vi "ConvertTextBasedCodeToLabVIEW.vi"() -> ()   [LabVIEW 2020]
uses:
  String/GDSString_ClassDescriptionType.ctl
  String/GDSString_AccessScopeModifierType.ctl
  String/GDSString_ModifierType.ctl
  String/GDSString_MethodDescriptionType.ctl
  CommonVIs/CommonVIs_AttributeType.ctl
  CommonVIs/CommonVIs_AttributeDataType.ctl
  CommonVIs/CommonVIs_PropertyType.ctl
  String/GDSString_ClassParentType.ctl
  String/GDSString_ClassType.ctl
  String/GDSString_ClassOwnerType.ctl
  CommonVIs/CommonVIs_EnumType.ctl
  CommonVIs/CommonVIs_StructType.ctl
  API/GDSAPI_SubVIs/GDSAPI_PropertyMethodType.ctl
  ScriptingFunctions/Scripting_ConnectorPanePatternType.ctl
  ConvertTextToLv_SubVIs/ConvertTextBasedCodeToLabVIEW_MissingType.ctl
  ConvertTextToLv_SubVIs/ConvertTextBasedCodeToLabVIEW_MissingTypeIconType.ctl
  <vilib>/picture/picture.llb/imagedata.ctl
  <vilib>/Utility/miscctls.llb/LVFontTypeDef.ctl
  <vilib>/Utility/miscctls.llb/LVBoundsTypeDef.ctl
  ConvertTextToLv_SubVIs/ConvertTextBasedCodeToLabVIEW_CreateClassesOption.ctl
  API/GDSAPI_SubVIs/GDSAPI_ClassProviderType.ctl
  <vilib>/Utility/miscctls.llb/LVPositionTypeDef.ctl
  <vilib>/Platform/browser.llb/Open URL in Default Browser (path).vi
  <vilib>/Utility/miscctls.llb/LVPointTypeDef.ctl
panel:
  out "Classes":T1[](array[typedef])
  out "Tab":T13(tab)
  in  "RemoveSelectedFiles":bool
  in  "ClearList":bool
  in  "FileList":i32[](listbox) caption="File List"
  in  "CopyfromClipboard":bool
  in  "Code":string caption="Java or C# Code"
  in  "Path":path caption="Java or C# File or top level folder"
  out "FileListText":bool
  in  "Ring":u16(ring)=2 items=["Select action to handle missing type", "Create stub code as class", "Create stub code as interface", "Remove dependency to this type"]
  out "Picture":picture caption="Missing Classes and types"
  in  "ExistingClasses":path
  out "MissingText1":string
  out "MissingText2":string
  in  "BetterNames":bool
  in  "ViewClassOverView":bool
  in  "ClassType":T14(ring) caption="Class Type"
  in  "Top Folder for all classes":path caption="Folder will be created"
  in  "PropertyMethodType":T15 caption="Property Method Type"
  in  "VI/Method Pattern type":T16 items=["4x4x4", "5x6x5", "6x8x6"]
  out "ProgressText":string
  in  "Previous":bool
  in  "Cancel":bool
  in  "Next":bool
  out "error IO":errorcluster
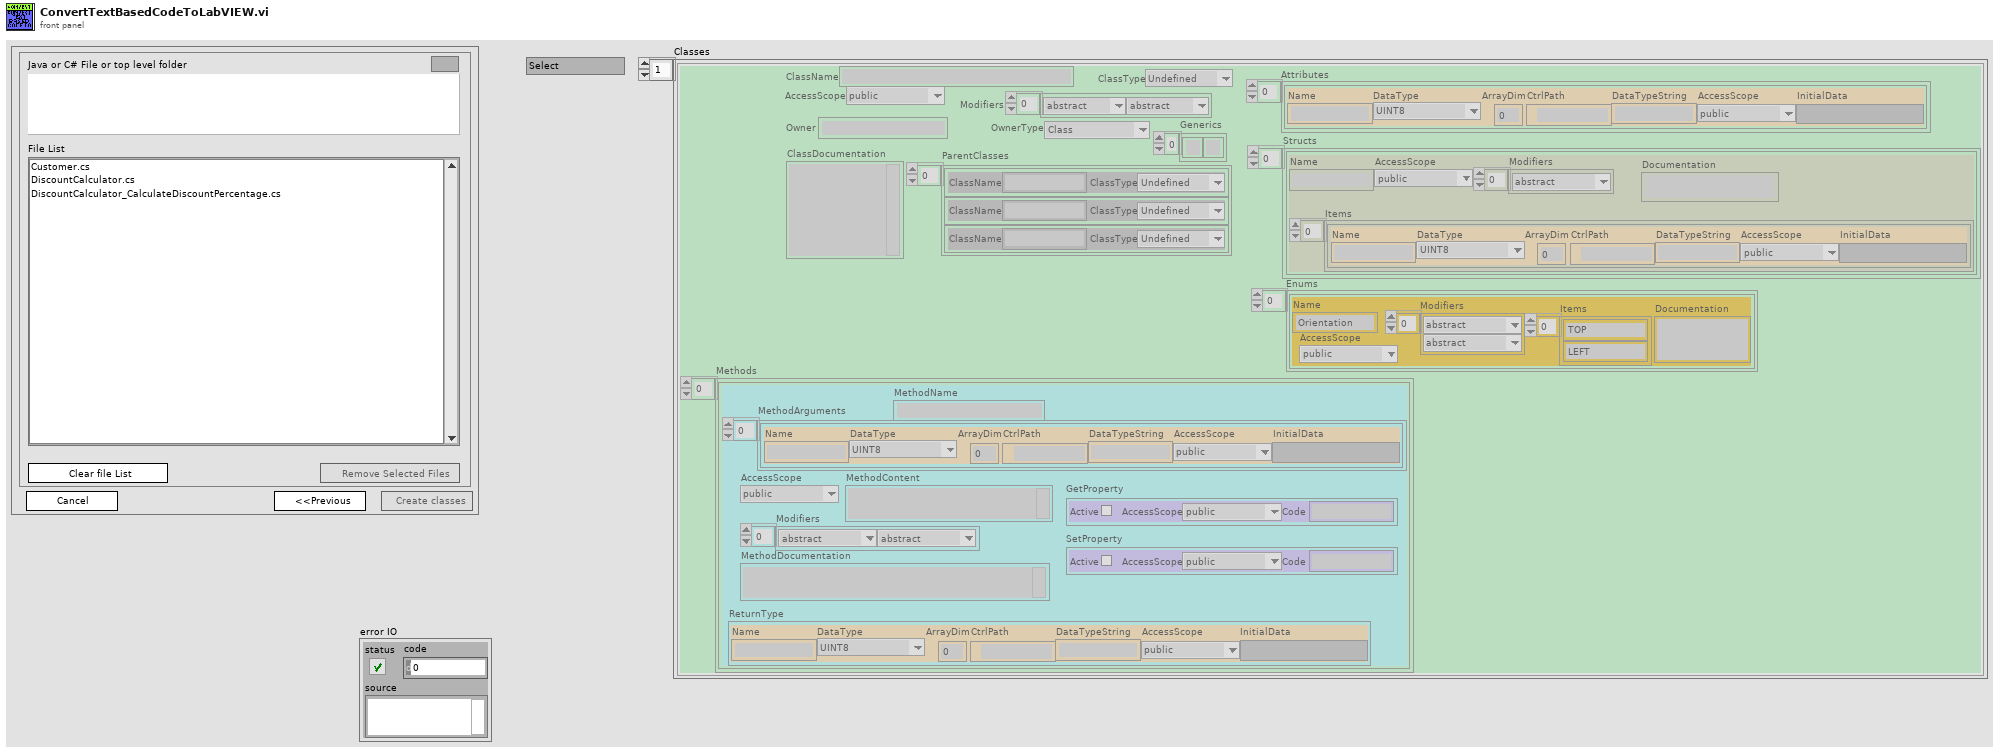
[diagram p1: front panel]
types:
  T1 = typedef "GDSString_ClassDescriptionType.ctl" = cluster{"ClassName":string, "AccessScope":T2, "Modifiers":T3[], "ClassDocumentation":string, "Methods":T4[], "ParentClasses":T8[], "ClassType":T9, "Owner":string, "OwnerType":T10, "Generics":string[], "Attributes":T5[], "Enums":T11[], "Structs":T12[]}
  T2 = typedef "GDSString_AccessScopeModifierType.ctl" = enum16{"public", "private", "protected", "internal"}
  T3 = typedef "GDSString_ModifierType.ctl" = enum16{"abstract", "static", "final", "synchronized", "strictfp", "async", "const", "event", "extern", "new", "native ", "override", "partial", "readonly", "sealed", "unsafe", "virtual", "volatile"}
  T4 = typedef "GDSString_MethodDescriptionType.ctl" = cluster{"ReturnType":T5, "MethodName":string, "AccessScope":T2, "Modifiers":T3[], "MethodDocumentation":string, "MethodContent":string, "MethodArguments":T5[], "GetProperty":T7, "SetProperty":T7}
  T5 = typedef "CommonVIs_AttributeType.ctl" = cluster{"Name":string, "DataType":T6, "ArrayDim":i32, "CtrlPath":path, "DataTypeString":string, "AccessScope":T2, "InitialData":variant}
  T6 = typedef "CommonVIs_AttributeDataType.ctl" = enum16{"UINT8", "INT8", "UINT16", "INT16", "UINT32", "INT32", "UINT64", "INT64", "SGL", "DBL", "EXT", "CSG", "CDB", "CXT", "TimeStamp", "STRING", "PATH", "BOOL", "ENUM", "RefNum", "VIRefNum", "LabVIEW Class", "Cluster", "Variant", "TypeDef", "Waveform", "LabVIEW Object", "Other", "void", "Set", "Map"}
  T7 = typedef "CommonVIs_PropertyType.ctl" = cluster{"Active":bool, "AccessScope":T2, "Code":string}
  T8 = typedef "GDSString_ClassParentType.ctl" = cluster{"ClassName":string, "ClassType":T9}
  T9 = typedef "GDSString_ClassType.ctl" = enum16{"Undefined", "Class", "Interface"}
  T10 = typedef "GDSString_ClassOwnerType.ctl" = enum16{"NoOwner", "Class", "Package/NameSpace"}
  T11 = typedef "CommonVIs_EnumType.ctl" = cluster{"Name":string, "AccessScope":T2, "Modifiers":T3[], "Items":string[], "Documentation":string}
  T12 = typedef "CommonVIs_StructType.ctl" = cluster{"Name":string, "AccessScope":T2, "Modifiers":T3[], "Items":T5[], "Documentation":string}
  T13 = enum32{"Select", "Analysing", "Missing", "Overview", "Working"}
  T14 = enum16{"Native By Value LabVIEW Classes", "Reference Object DVR (GOOP4)", "Reference Object  (GOOP3)"}
  T15 = typedef "GDSAPI_PropertyMethodType.ctl" = enum16{"PropertyMethod", "PropertyNode"}
  T16 = typedef "Scripting_ConnectorPanePatternType.ctl" = u16
  T17 = typedef "imagedata.ctl" = cluster{"image type":i32, "image depth":i32, "image":u8[], "mask":u8[], "colors":u32[], "Rectangle":cluster{"left":i16, "top":i16, "right":i16, "bottom":i16}}
  T18 = typedef "ConvertTextBasedCodeToLabVIEW_MissingType.ctl" = cluster{"Item":string, "Options":string[], "Icons":T19[], "Index":i32}
  T19 = typedef "ConvertTextBasedCodeToLabVIEW_MissingTypeIconType.ctl" = enum16{"?", "Add", "Delete", "Implement", "Inherit"}
  T20 = cluster{"Counter":i32, "Text":string, "Cancelled":bool, "Files":path[], "Classes":T1[], "MissingTypes":cluster{"ShowRing":bool, "Rectangle":cluster{"left":i16, "top":i16, "right":i16, "bottom":i16}, "IndexOffset":i32, "Row":i32, "Y-Distance":i32, "Selected":i32[], "Font":enum16{"User-specified Font", "Application Font", "System Font", "Dialog Font"}, "UserFont":cluster{"Font Name:":string, "Size":i16, "Strikeout?":bool, "Italic?":bool, "Underline?":bool, "Outline?":bool, "Shadow?":bool, "Bold?":bool}, "VerGap":i32, "HorGap":i32, "XStart2":i32, "XStart1":i32, "Rectangles":cluster{"left":i16, "top":i16, "right":i16, "bottom":i16}[], "VerticalRows":i32, "YStart":i32}, "MissingItems":T18[], "ExistingClassesFolders":path[], "StructsOusideClass":T12[], "EnumsOusideClass":T11[], "InterfaceItems":T18[], "Interface":bool, "MissingTypeSelected":i32[], "InterfaceSelected":i32[]}
  T21 = typedef "LVPointTypeDef.ctl" = cluster{"Horizontal":i16, "Vertical":i16}
  T22 = enum8{"Enabled", "Disabled", "Disabled and Grayed Out"}
  T23 = enum32{"Select", "Analysing", "Missing", "Overview"}
  T24 = typedef "LVFontTypeDef.ctl" = cluster{"Font Name":string, "Size":u16, "Bold":bool, "Italic":bool, "Underline":bool, "Strikeout":bool, "Color":u32}
  T25 = cluster{"left":i16, "top":i16, "right":i16, "bottom":i16}
  T26 = typedef "LVBoundsTypeDef.ctl" = cluster{"Width":u32, "Height":u32}
  T27 = typedef "ConvertTextBasedCodeToLabVIEW_CreateClassesOption.ctl" = cluster{"ClassProvider":T28, "PropertyMethodType":T15, "Pattern type":T16}
  T28 = typedef "GDSAPI_ClassProviderType.ctl" = enum16{"LabVIEW Native(By value)", "GOOP-3(By reference)", "GOOP-4(By reference)"}
  T29 = typedef "LVMouseTypeDef.ctl" = cluster{"Mouse Position":cluster{"X":i32, "Y":i32}, "Mouse Modifiers":cluster{"Button Down":bool, "Shift Mod":bool, "Menu Mod":bool, "Option Mod":bool}}
  T30 = cluster{"left":i16, "top":i16, "right":i16, "bottom":i16}[]
  T31 = cluster{"Font Name:":string, "Size":i16, "Strikeout?":bool, "Italic?":bool, "Underline?":bool, "Outline?":bool, "Shadow?":bool, "Bold?":bool}
  T32 = enum16{"User-specified Font", "Application Font", "System Font", "Dialog Font"}
  T33 = typedef "LVRectTypeDef.ctl" = cluster{"Left":i16, "Top":i16, "Right":i16, "Bottom":i16}
  T34 = typedef "LVPositionTypeDef.ctl" = cluster{"Left":i32, "Top":i32}
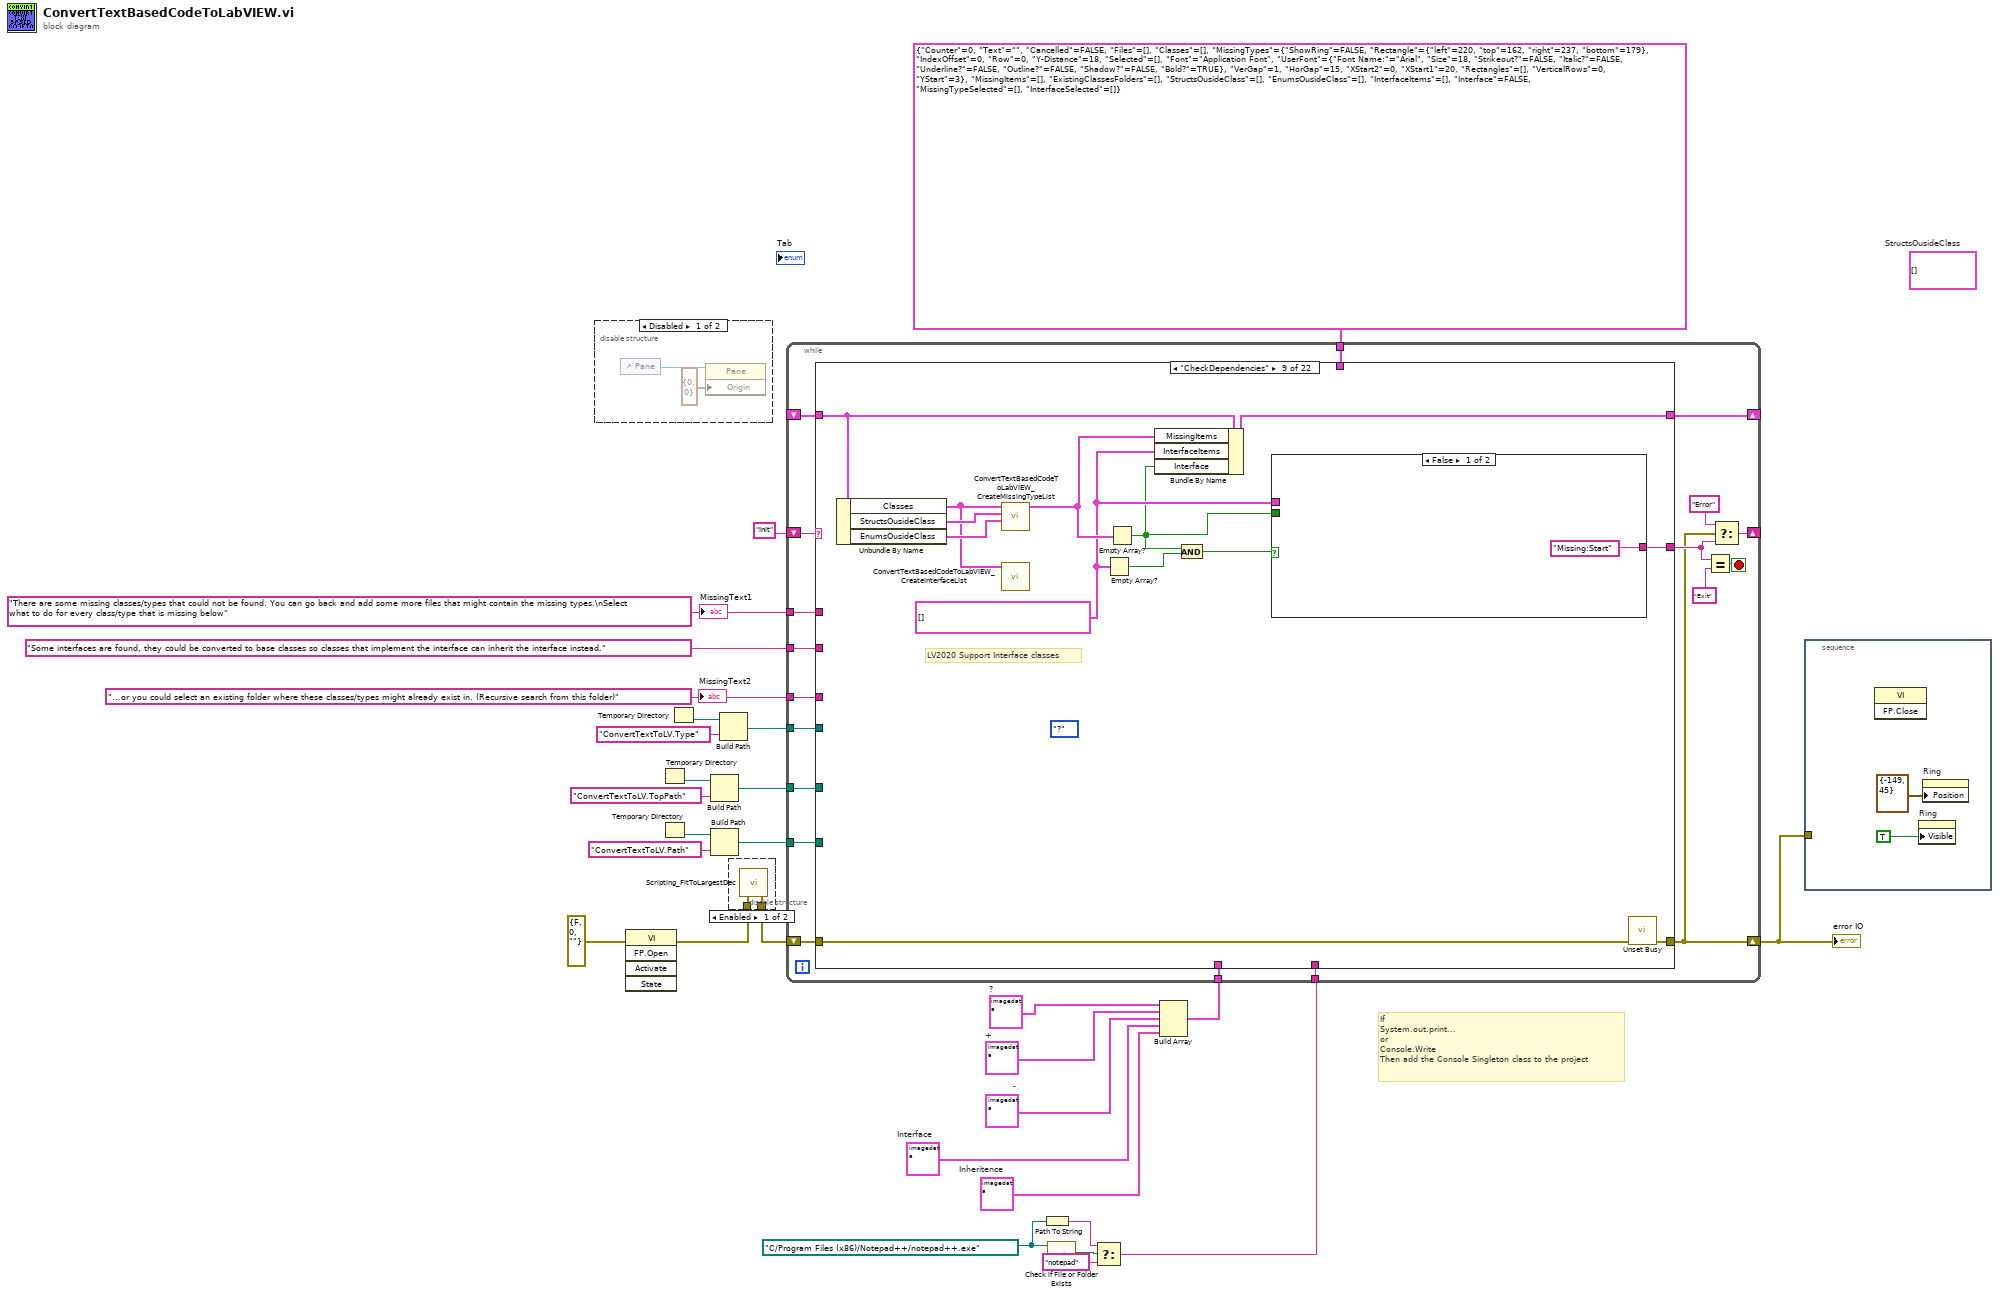
[diagram p0: block diagram]
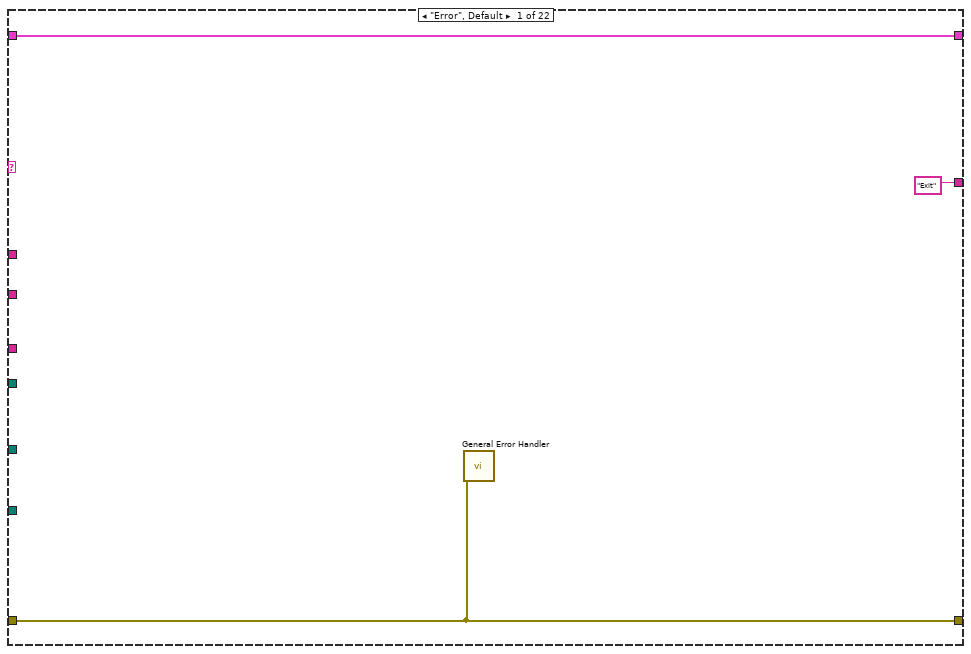
[diagram p4: hidden frame]
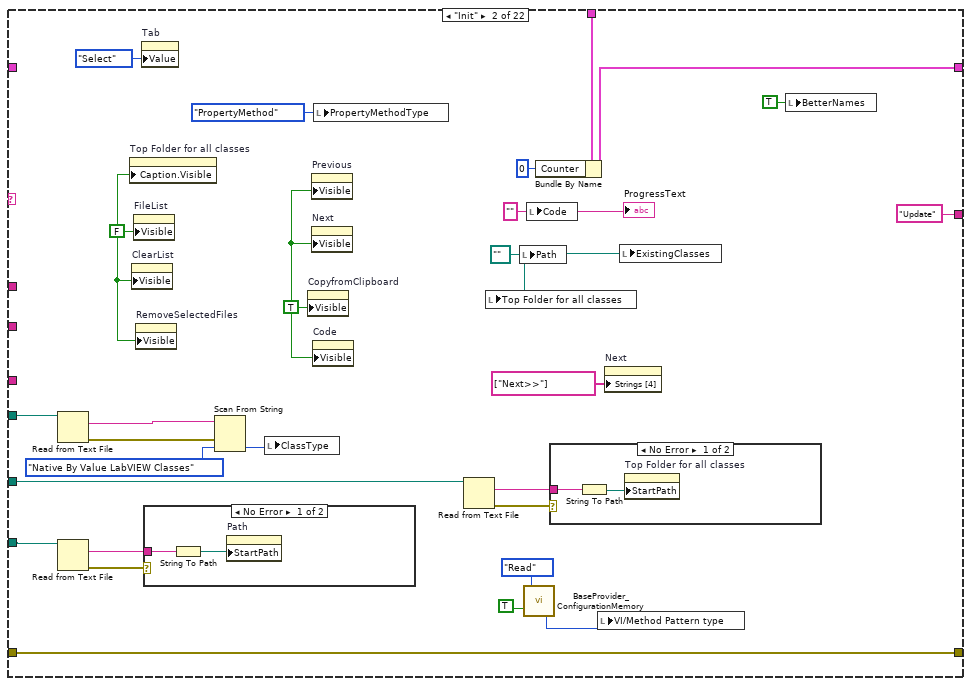
[diagram p5: hidden frame]
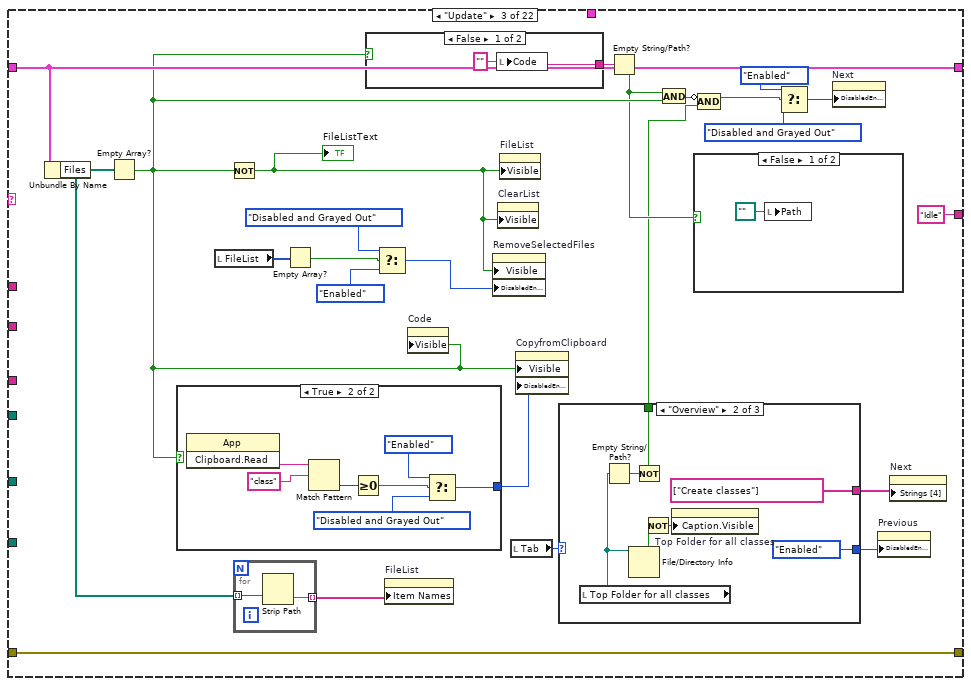
[diagram p8: hidden frame]
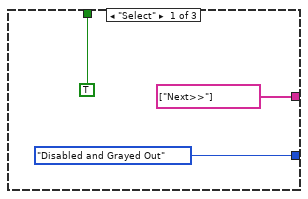
[diagram p9: hidden frame]
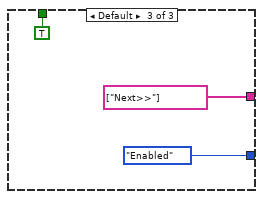
[diagram p10: hidden frame]
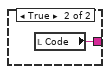
[diagram p12: hidden frame]
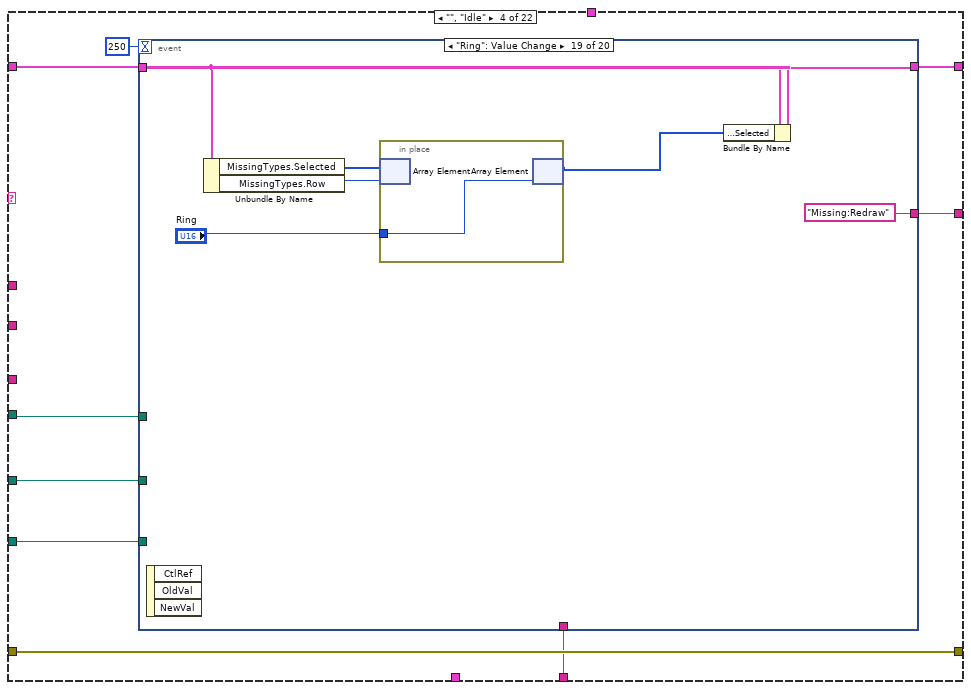
[diagram p14: hidden frame]
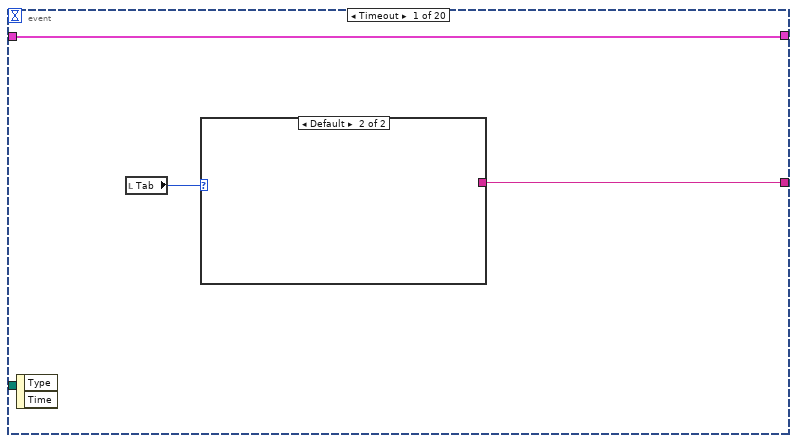
[diagram p15: hidden frame]
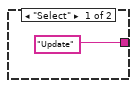
[diagram p16: hidden frame]
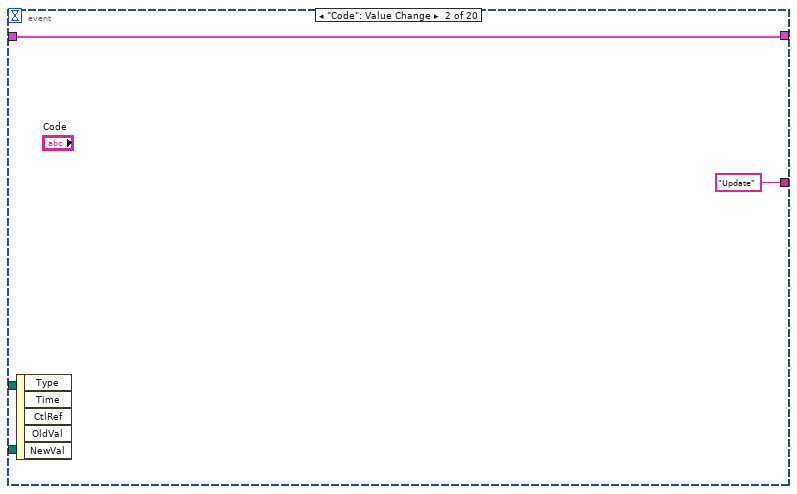
[diagram p17: hidden frame]
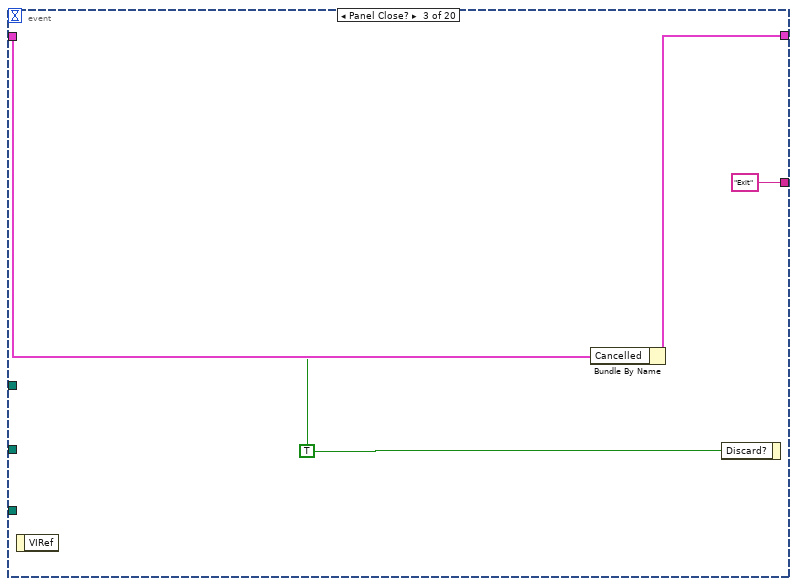
[diagram p18: hidden frame]
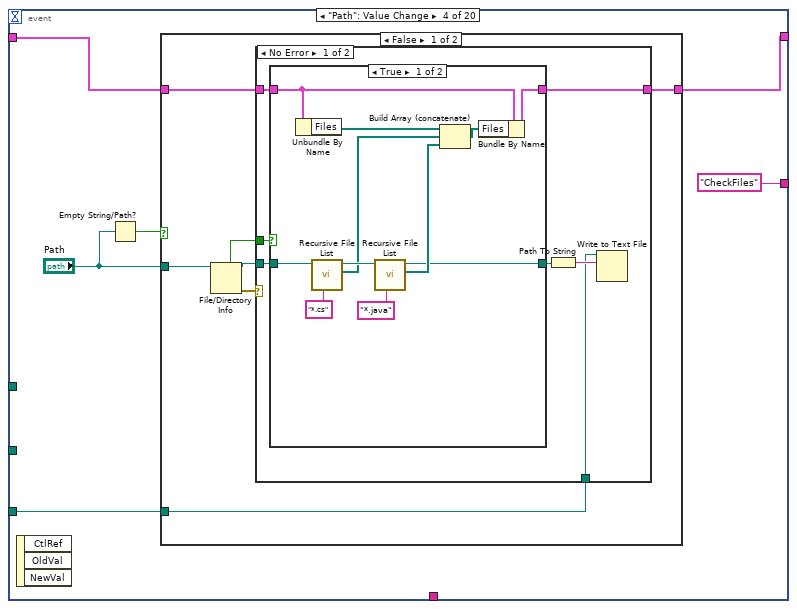
[diagram p19: hidden frame]
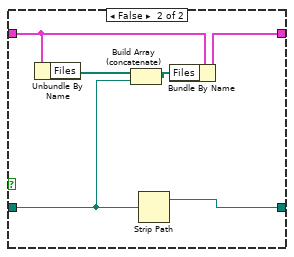
[diagram p20: hidden frame]
diagram:
  w1 = T17 {"image type"=0, "image depth"=32, "image"=array[1024 elements], "mask"=[255, 255, 255, 255, 255, 255, 255, 255, 255, 255, 255, 255, 255, 255, 255, 255, 255, 255, 255, 255, 255, 255, 255, 255, 255, 255, 255, 255, 255, 255, 255, 255], "colors"=[], "Rectangle"={"left"=0, "top"=0, "right"=16, "bottom"=16}}  # Inheritence
  w2 = T17 {"image type"=0, "image depth"=32, "image"=array[1024 elements], "mask"=[255, 255, 255, 255, 255, 255, 255, 255, 255, 255, 255, 255, 255, 255, 255, 255, 255, 255, 255, 255, 255, 255, 255, 255, 255, 255, 255, 255, 255, 255, 255, 255], "colors"=[], "Rectangle"={"left"=0, "top"=0, "right"=16, "bottom"=16}}  # Interface
  w4 = "...or you could select an existing folder where these classes/types might already exist in. (Recursive search from this folder)" ("MissingText2")
  w5 = "There are some missing classes/types that could not be found. You can go back and add some more files that might contain the missing types.\nSelect what to do for every class/type that is missing below" ("MissingText")
  (unwired) T12[] []  # StructsOusideClass
  w17 = T17 {"image type"=0, "image depth"=32, "image"=array[1024 elements], "mask"=[0, 0, 15, 224, 63, 248, 127, 252, 127, 252, 255, 254, 255, 254, 255, 254, 255, 254, 255, 254, 255, 254, 255, 254, 127, 252, 127, 252, 63, 248, 15, 224], "colors"=[], "Rectangle"={"left"=0, "top"=0, "right"=16, "bottom"=16}}  # ?
  w15 = T17 {"image type"=0, "image depth"=32, "image"=[0, 0, 0, 0, 0, 0, 0, 0, 78, 142, 77, 90, 2, 148, 148, 147, 0, 0, 0, 0, 0, 0, 0, 0, 0, 0, 0, 0, 0, 0, 0, 0, 0, 0, 0, 0, 0, 0, 0, 0, 0, 0, 0, 0, 48, 145, 103, 111, 3, 148, 145, 146, 0, 0, 0, 0, 0, 0, 0, 0, 0, 0, 0, 0, 0, 0, 0, 0, 113, 246, 155, 172, 255, 238, 54, 90, 164, 243, 121, 144, 0, 0, 0, 0, 0, 0, 0, 0, 0, 0, 0, 0, 0, 0, 0, 0, 0, 0, 0, 0, 0, 0, 0, 0, 114, 247, 158, 175, 255, 238, 55, 91, 247, 238, 61, 95, 190, 242, 101, 128, 55, 251, 205, 215, 0, 0, 0, 0, 37, 251, 214, 220, 252, 236, 52, 88, 255, 237, 57, 92, 255, 235, 54, 90, 150, 242, 130, 151, 0, 0, 0, 0, 0, 0, 0, 0, 0, 0, 0, 0, 0, 0, 0, 0, 64, 249, 199, 209, 253, 236, 55, 90, 254, 235, 56, 91, 255, 236, 54, 90, 127, 244, 146, 165, 0, 0, 0, 0, 0, 0, 0, 0, 0, 0, 0, 0, 64, 249, 193, 203, 240, 236, 60, 95, 255, 237, 57, 92, 255, 236, 55, 90, 136, 243, 141, 161, 0, 0, 0, 0, 0, 0, 0, 0, 25, 252, 231, 235, 235, 237, 66, 99, 255, 236, 57, 92, 255, 236, 54, 90, 118, 244, 150, 168, 0, 0, 0, 0, 0, 0, 0, 0, 0, 0, 0, 0, 0, 0, 0, 0, 0, 0, 0, 0, 39, 251, 215, 222, 224, 237, 70, 103, 255, 236, 57, 92, 255, 235, 53, 89, 121, 244, 152, 170, 1, 254, 253, 254, 201, 239, 91, 120, 254, 235, 56, 91, 255, 236, 55, 90, 121, 244, 150, 168, 0, 0, 0, 0, 0, 0, 0, 0, 0, 0, 0, 0, 0, 0, 0, 0, 0, 0, 0, 0, 0, 0, 0, 0, 0, 0, 0, 0, 20, 252, 233, 236, 204, 238, 86, 115, 255, 236, 57, 92, 255, 236, 55, 91, 194, 239, 93, 122, 255, 236, 56, 92, 255, 236, 55, 90, 133, 243, 143, 163, 0, 0, 0, 0, 0, 0, 0, 0, 0, 0, 0, 0, 0, 0, 0, 0, 0, 0, 0, 0, 0, 0, 0, 0, 0, 0, 0, 0, 0, 0, 0, 0, 0, 0, 0, 0, 12, 253, 243, 245, 210, 238, 83, 114, 255, 236, 57, 92, 254, 235, 56, 91, 255, 236, 56, 92, 149, 242, 132, 153, 0, 0, 0, 0, 0, 0, 0, 0, 0, 0, 0, 0, 0, 0, 0, 0, 0, 0, 0, 0, 0, 0, 0, 0, 0, 0, 0, 0, 0, 0, 0, 0, 0, 0, 0, 0, 0, 0, 0, 0, 0, 0, 0, 0, 78, 248, 186, 198, 255, 236, 55, 91, 255, 237, 58, 93, 253, 236, 55, 90, 39, 251, 220, 226, 0, 0, 0, 0, 0, 0, 0, 0, 0, 0, 0, 0, 0, 0, 0, 0, 0, 0, 0, 0, 0, 0, 0, 0, 0, 0, 0, 0, 0, 0, 0, 0, 0, 0, 0, 0, 0, 0, 0, 0, 11, 253, 244, 245, 222, 237, 74, 105, 254, 236, 56, 92, 253, 236, 56, 91, 255, 236, 57, 92, 210, 238, 85, 116, 5, 254, 250, 250, 0, 0, 0, 0, 0, 0, 0, 0, 0, 0, 0, 0, 0, 0, 0, 0, 0, 0, 0, 0, 0, 0, 0, 0, 0, 0, 0, 0, 0, 0, 0, 0, 0, 0, 0, 0, 167, 241, 117, 142, 255, 236, 55, 91, 179, 240, 108, 134, 139, 244, 138, 159, 255, 236, 56, 91, 255, 236, 56, 91, 147, 243, 132, 153, 0, 0, 0, 0, 0, 0, 0, 0, 0, 0, 0, 0, 0, 0, 0, 0, 0, 0, 0, 0, 0, 0, 0, 0, 0, 0, 0, 0, 0, 0, 0, 0, 100, 247, 169, 184, 255, 236, 55, 90, 255, 235, 54, 90, 54, 250, 206, 215, 6, 253, 248, 249, 227, 237, 71, 103, 254, 235, 56, 91, 255, 236, 54, 90, 77, 248, 188, 200, 0, 0, 0, 0, 0, 0, 0, 0, 0, 0, 0, 0, 0, 0, 0, 0, 0, 0, 0, 0, 0, 0, 0, 0, 40, 251, 219, 224, 247, 236, 57, 92, 255, 236, 57, 92, 185, 240, 103, 129, 0, 0, 0, 0, 0, 0, 0, 0, 100, 246, 164, 180, 255, 236, 56, 91, 255, 236, 57, 92, 238, 237, 64, 98, 25, 252, 232, 236, 0, 0, 0, 0, 0, 0, 0, 0, 0, 0, 0, 0, 0, 0, 0, 0, 4, 254, 250, 251, 211, 238, 83, 113, 254, 235, 56, 91, 255, 236, 54, 90, 56, 250, 206, 214, 0, 0, 0, 0, 0, 0, 0, 0, 4, 254, 247, 249, 228, 237, 68, 100, 255, 237, 57, 92, 254, 235, 56, 91, 193, 239, 96, 125, 0, 0, 0, 0, 0, 0, 0, 0, 0, 0, 0, 0, 0, 0, 0, 0, 139, 244, 137, 157, 255, 237, 55, 91, 255, 237, 56, 92, 188, 229, 93, 119, 0, 0, 0, 0, 0, 0, 0, 0, 0, 0, 0, 0, 0, 0, 0, 0, 105, 246, 160, 177, 255, 236, 55, 90, 255, 236, 56, 92, 255, 236, 54, 90, 127, 244, 148, 166, 0, 0, 0, 0, 0, 0, 0, 0, 26, 246, 224, 228, 199, 228, 84, 112, 200, 227, 87, 114, 201, 227, 85, 113, 57, 237, 196, 204, 0, 0, 0, 0, 0, 0, 0, 0, 0, 0, 0, 0, 0, 0, 0, 0, 7, 254, 247, 249, 171, 231, 108, 133, 170, 241, 120, 144, 167, 239, 120, 143, 162, 235, 117, 140, 17, 241, 227, 230, 0, 0, 0, 0, 0, 0, 0, 0, 0, 0, 0, 0, 0, 0, 0, 0, 0, 0, 0, 0, 0, 0, 0, 0, 0, 0, 0, 0, 0, 0, 0, 0, 0, 0, 0, 0, 0, 0, 0, 0, 0, 0, 0, 0, 0, 0, 0, 0, 0, 0, 0, 0, 0, 0, 0, 0, 0, 0, 0, 0, 0, 0, 0, 0, 0, 0, 0, 0], "mask"=[0, 0, 48, 28, 120, 60, 60, 112, 28, 224, 15, 224, 7, 192, 3, 128, 7, 192, 15, 224, 12, 224, 28, 112, 56, 120, 120, 60, 112, 60, 0, 0], "colors"=[], "Rectangle"={"left"=0, "top"=0, "right"=16, "bottom"=16}}  # -
  w16 = T17 {"image type"=0, "image depth"=32, "image"=[0, 0, 0, 0, 0, 0, 0, 0, 0, 0, 0, 0, 0, 0, 0, 0, 0, 0, 0, 0, 255, 0, 173, 0, 255, 0, 173, 0, 255, 0, 173, 0, 255, 0, 173, 0, 255, 0, 173, 0, 0, 0, 0, 0, 0, 0, 0, 0, 0, 0, 0, 0, 0, 0, 0, 0, 0, 0, 0, 0, 0, 0, 0, 0, 0, 0, 0, 0, 0, 0, 0, 0, 0, 0, 0, 0, 0, 0, 0, 0, 0, 0, 0, 0, 255, 0, 173, 0, 255, 0, 173, 0, 255, 0, 173, 0, 255, 0, 173, 0, 255, 0, 173, 0, 255, 106, 100, 106, 0, 0, 0, 0, 0, 0, 0, 0, 0, 0, 0, 0, 0, 0, 0, 0, 0, 0, 0, 0, 0, 0, 0, 0, 0, 0, 0, 0, 0, 0, 0, 0, 0, 0, 0, 0, 0, 0, 0, 0, 255, 0, 173, 0, 255, 0, 173, 0, 255, 0, 173, 0, 255, 0, 173, 0, 255, 0, 173, 0, 255, 106, 100, 106, 0, 0, 0, 0, 0, 0, 0, 0, 0, 0, 0, 0, 0, 0, 0, 0, 0, 0, 0, 0, 0, 0, 0, 0, 0, 0, 0, 0, 0, 0, 0, 0, 0, 0, 0, 0, 0, 0, 0, 0, 255, 0, 173, 0, 255, 0, 173, 0, 255, 0, 173, 0, 255, 0, 173, 0, 255, 0, 173, 0, 255, 106, 100, 106, 0, 0, 0, 0, 0, 0, 0, 0, 0, 0, 0, 0, 0, 0, 0, 0, 0, 0, 0, 0, 0, 0, 0, 0, 0, 0, 0, 0, 0, 0, 0, 0, 0, 0, 0, 0, 0, 0, 0, 0, 255, 0, 173, 0, 255, 0, 173, 0, 255, 0, 173, 0, 255, 0, 173, 0, 255, 0, 173, 0, 255, 106, 100, 106, 0, 0, 0, 0, 0, 0, 0, 0, 0, 0, 0, 0, 0, 0, 0, 0, 0, 0, 0, 0, 255, 0, 173, 0, 255, 0, 173, 0, 255, 0, 173, 0, 255, 0, 173, 0, 255, 0, 173, 0, 255, 0, 173, 0, 255, 0, 173, 0, 255, 0, 173, 0, 255, 0, 173, 0, 255, 0, 173, 0, 255, 0, 173, 0, 255, 0, 173, 0, 255, 0, 173, 0, 255, 0, 173, 0, 255, 0, 173, 0, 0, 0, 0, 0, 255, 0, 173, 0, 255, 0, 173, 0, 255, 0, 173, 0, 255, 0, 173, 0, 255, 0, 173, 0, 255, 0, 173, 0, 255, 0, 173, 0, 255, 0, 173, 0, 255, 0, 173, 0, 255, 0, 173, 0, 255, 0, 173, 0, 255, 0, 173, 0, 255, 0, 173, 0, 255, 0, 173, 0, 255, 0, 173, 0, 255, 106, 100, 106, 255, 0, 173, 0, 255, 0, 173, 0, 255, 0, 173, 0, 255, 0, 173, 0, 255, 0, 173, 0, 255, 0, 173, 0, 255, 0, 173, 0, 255, 0, 173, 0, 255, 0, 173, 0, 255, 0, 173, 0, 255, 0, 173, 0, 255, 0, 173, 0, 255, 0, 173, 0, 255, 0, 173, 0, 255, 0, 173, 0, 255, 106, 100, 106, 255, 0, 173, 0, 255, 0, 173, 0, 255, 0, 173, 0, 255, 0, 173, 0, 255, 0, 173, 0, 255, 0, 173, 0, 255, 0, 173, 0, 255, 0, 173, 0, 255, 0, 173, 0, 255, 0, 173, 0, 255, 0, 173, 0, 255, 0, 173, 0, 255, 0, 173, 0, 255, 0, 173, 0, 255, 0, 173, 0, 255, 106, 100, 106, 255, 0, 173, 0, 255, 0, 173, 0, 255, 0, 173, 0, 255, 0, 173, 0, 255, 0, 173, 0, 255, 0, 173, 0, 255, 0, 173, 0, 255, 0, 173, 0, 255, 0, 173, 0, 255, 0, 173, 0, 255, 0, 173, 0, 255, 0, 173, 0, 255, 0, 173, 0, 255, 0, 173, 0, 255, 0, 173, 0, 255, 106, 100, 106, 0, 0, 0, 0, 255, 106, 100, 106, 255, 106, 100, 106, 255, 106, 100, 106, 255, 106, 100, 106, 255, 0, 173, 0, 255, 0, 173, 0, 255, 0, 173, 0, 255, 0, 173, 0, 255, 0, 173, 0, 255, 106, 100, 106, 255, 106, 100, 106, 255, 106, 100, 106, 255, 106, 100, 106, 255, 106, 100, 106, 255, 106, 100, 106, 0, 0, 0, 0, 0, 0, 0, 0, 0, 0, 0, 0, 0, 0, 0, 0, 0, 0, 0, 0, 255, 0, 173, 0, 255, 0, 173, 0, 255, 0, 173, 0, 255, 0, 173, 0, 255, 0, 173, 0, 255, 106, 100, 106, 0, 0, 0, 0, 0, 0, 0, 0, 0, 0, 0, 0, 0, 0, 0, 0, 0, 0, 0, 0, 0, 0, 0, 0, 0, 0, 0, 0, 0, 0, 0, 0, 0, 0, 0, 0, 0, 0, 0, 0, 255, 0, 173, 0, 255, 0, 173, 0, 255, 0, 173, 0, 255, 0, 173, 0, 255, 0, 173, 0, 255, 106, 100, 106, 0, 0, 0, 0, 0, 0, 0, 0, 0, 0, 0, 0, 0, 0, 0, 0, 0, 0, 0, 0, 0, 0, 0, 0, 0, 0, 0, 0, 0, 0, 0, 0, 0, 0, 0, 0, 0, 0, 0, 0, 255, 0, 173, 0, 255, 0, 173, 0, 255, 0, 173, 0, 255, 0, 173, 0, 255, 0, 173, 0, 255, 106, 100, 106, 0, 0, 0, 0, 0, 0, 0, 0, 0, 0, 0, 0, 0, 0, 0, 0, 0, 0, 0, 0, 0, 0, 0, 0, 0, 0, 0, 0, 0, 0, 0, 0, 0, 0, 0, 0, 0, 0, 0, 0, 255, 0, 173, 0, 255, 0, 173, 0, 255, 0, 173, 0, 255, 0, 173, 0, 255, 0, 173, 0, 255, 106, 100, 106, 0, 0, 0, 0, 0, 0, 0, 0, 0, 0, 0, 0, 0, 0, 0, 0, 0, 0, 0, 0, 0, 0, 0, 0, 0, 0, 0, 0, 0, 0, 0, 0, 0, 0, 0, 0, 0, 0, 0, 0, 0, 0, 0, 0, 255, 106, 100, 106, 255, 106, 100, 106, 255, 106, 100, 106, 255, 106, 100, 106, 255, 106, 100, 106, 0, 0, 0, 0, 0, 0, 0, 0, 0, 0, 0, 0, 0, 0, 0, 0, 0, 0, 0, 0], "mask"=[7, 192, 7, 224, 7, 224, 7, 224, 7, 224, 255, 254, 255, 255, 255, 255, 255, 255, 255, 255, 127, 255, 7, 224, 7, 224, 7, 224, 7, 224, 3, 224], "colors"=[], "Rectangle"={"left"=0, "top"=0, "right"=16, "bottom"=16}}  # +
  w21 = path "C:/Program Files (x86)/Notepad++/notepad++.exe"
  # "If\nSystem.out.print...\nor\nConsole.Write\nThen add the Console Singleton class to the project"
  n1 = disable-structure shown="Disabled" {
    frame Disabled {
      n2 = control-ref of="Pane"() -> (w30:refnum<vi>)
      n3 = property class="Pane"(reference=w30, "Origin"=T21 {"Horizontal"=0, "Vertical"=0}) -> ()  [unwired: 1 in, 2 out]
    }
    frame Enabled {
    }
  }
  n4 = invoke class="VI" method="FP.Open"(error in=errorcluster {"status"=FALSE, "code"=0, "source"=""} ("error IO")) -> (error out=w6:errorcluster)  [unwired: 4 in, 4 out]
  n5 = Temporary Directory() -> (w9:path)
  n6 = Temporary Directory() -> (w26:path)
  n7 = Temporary Directory() -> (w12:path)
  n8 = Build Path(base path=w9, name or relative path="ConvertTextToLV.TopPath") -> (appended path=w7:path)
  n9 = Build Path(base path=w26, name or relative path="ConvertTextToLV.Path") -> (appended path=w25:path)
  n10 = Build Path(base path=w12, name or relative path="ConvertTextToLV.Type") -> (appended path=w10:path)
  n11 = disable-structure shown="Enabled" {
    disable-tunnel: w6 -> [w33 _]
    disable-tunnel: [w32 _] -> w23
    frame Enabled {
      n12 = call "Scripting_FitToLargestDec.vi"("error in (no error)"=w33) -> ("error out"=w32:errorcluster)  [unwired: 5 in, 1 out]
    }
    frame Disabled {
    }
  }
  n13 = Path To String(path=w21) -> (string=w20:string)
  n14 = call <vilib>:"Check if File or Folder Exists.vi"("path"=w21) -> ("file or folder exists?"=w22:bool)  [unwired: 8 in, 2 out]
  n15 = Select(t=w20, s=w22, f="notepad") -> (s? t:f=w18:string)
  n16 = Build Array(w17, w16, w15, w2, w1) -> (w14:T17[])
  n17 = while {
    shift-right: [w45] -> w13
    shift-left: w23 -> [w52]
    shift-right: [w50] -> _
    shift-left: "Init" -> [w51]
    shift-right: [w44] -> _
    shift-left: _ -> [w43]
    tunnel: T20 {"Counter"=0, "Text"="", "Cancelled"=FALSE, "Files"=[], "Classes"=[], "MissingTypes"={"ShowRing"=FALSE, "Rectangle"={"left"=220, "top"=162, "right"=237, "bottom"=179}, "IndexOffset"=0, "Row"=0, "Y-Distance"=18, "Selected"=[], "Font"=enum."Application Font", "UserFont"={"Font Name:"="Arial", "Size"=18, "Strikeout?"=FALSE, "Italic?"=FALSE, "Underline?"=FALSE, "Outline?"=FALSE, "Shadow?"=FALSE, "Bold?"=TRUE}, "VerGap"=1, "HorGap"=15, "XStart2"=0, "XStart1"=20, "Rectangles"=[], "VerticalRows"=0, "YStart"=3}, "MissingItems"=[], "ExistingClassesFolders"=[], "StructsOusideClass"=[], "EnumsOusideClass"=[], "InterfaceItems"=[], "Interface"=FALSE, "MissingTypeSelected"=[], "InterfaceSelected"=[]} -> [w42]
    tunnel: w25 -> [w41]
    tunnel: w18 -> [w40]
    tunnel: w14 -> [w39]
    tunnel: w10 -> [w38]
    tunnel: w7 -> [w37]
    tunnel: w5 -> [w36]
    tunnel: w4 -> [w35]
    tunnel: "Some interfaces are found, they could be converted to base classes so classes that implement the interface can inherit the interface instead." ("MissingText") -> [w34]
    stop <- w49 stop-if-true
    n18 = case shown="\"CheckDependencies\"" w51 {
      tunnel: w52 -> [w53 w81 w108 w141 w399 w429 w464 w566 w577 w583 w597 w605 w675 w737 w776 w782 w793 w800 w802 w826 w866 w891]
      tunnel: [w53 w81 w108 w141 w398 w429 w464 w566 w578 w583 w597 w605 w675 w737 w776 w782 w793 w800 w802 w825 w865 w891] -> w45
      tunnel: ["Exit" "Update" "Idle" w142 w391 "ReplaceDataTypeOther" "FindGenericTypes" "CheckDependencies" w579 _ "Missing:Init" ("format string") "Missing:Redraw" ("format string") "Missing:EnableNext?" ("format string") "Idle" ("format string") _ "Idle" ("format string") _ _ "Update" "Idle" "Done" w883] -> w46
      tunnel: [w54 w80 w109 w143 w392 w431 w465 w563 w569 w584 w589 w604 w656 w724 w744 w779 w784 w801 w803 w830 w870 w890] -> w44
      tunnel: w43 -> [w54 _ w109 w144 w397 w432 w466 w564 w570 w584 w589 w602 w649 w725 w739 w778 w784 w801 w805 w830 w870 w890]
      tunnel: w42 -> [_ w78 _ _ _ _ _ _ _ _ _ _ _ _ _ _ _ _ _ _ _ _]
      tunnel: w41 -> [_ w77 _ w140 _ _ _ _ _ _ _ _ _ _ _ _ _ _ _ _ _ _]
      tunnel: w40 -> [_ _ _ w139 _ _ _ _ _ _ _ _ _ _ _ _ _ _ _ _ _ _]
      tunnel: w39 -> [_ _ _ _ _ _ _ _ _ _ _ _ w654 _ _ _ _ _ _ _ _ _]
      tunnel: w38 -> [_ w71 _ w138 _ _ _ _ _ _ _ _ _ _ _ _ _ _ _ _ _ _]
      tunnel: w37 -> [_ w62 _ w137 _ _ _ _ _ _ _ _ _ _ _ _ _ _ _ _ _ _]
      tunnel: w36 -> [_ _ _ _ _ _ _ _ _ _ w587 _ _ _ _ _ _ _ _ _ _ _]
      tunnel: w35 -> [_ _ _ _ _ _ _ _ _ _ w585 _ _ _ _ _ _ _ _ _ _ _]
      tunnel: w34 -> [_ _ _ _ _ _ _ _ _ _ w586 _ _ _ _ _ _ _ _ _ _ _]
      frame "Error", Default {
        n19 = call <vilib>:"General Error Handler.vi"("error in (no error)"=w53) -> ()  [unwired: 10 in, 5 out]
      }
      frame "Init" {
        w65 = TRUE ("Visible")
        w73 = path "" ("Path")
        w66 = "" ("Code")
        w57 = FALSE ("Visible")
        n20 = Read from Text File(file (use dialog)=w71) -> (text=w72:string, error out=w68:errorcluster)  [unwired: 3 in, 2 out]
        n21 = Read from Text File(file (use dialog)=w77) -> (text=w75:string, error out=w76:errorcluster)  [unwired: 3 in, 2 out]
        n22 = property on="Top Folder for all classes" class="Path"("Caption.Visible"=w57) -> ()  [unwired: 2 in, 2 out]
        n23 = property on="ClearList" class="Bool"("Visible"=w57) -> ()  [unwired: 2 in, 2 out]
        n24 = property on="FileList" class="LstBox (strict)"("Visible"=w57) -> ()  [unwired: 2 in, 2 out]
        n25 = property on="RemoveSelectedFiles" class="Bool"("Visible"=w57) -> ()  [unwired: 2 in, 2 out]
        n26 = property on="Tab" class="TabCtl (strict)"("Value"=T13."Select" ("Tab")) -> ()  [unwired: 2 in, 2 out]
        n27 = case shown="No Error" w76 {
          tunnel: w75 -> [w86 _]
          frame No Error {
            n28 = String To Path(string=w86) -> (path=w85:path)
            n29 = property on="Path" class="Path"("StartPath"=w85) -> ()  [unwired: 2 in, 2 out]
          }
          frame Error {
          }
        }
        n30 = Scan From String(input string=w72, error in=w68, default 1=T14."Native By Value LabVIEW Classes" ("ClassType")) -> (output 1=w69:T14)  [unwired: 2 in, 3 out]
        n31 = local write "ClassType"(w69) -> ()
        n32 = property on="CopyfromClipboard" class="Bool"("Visible"=w65) -> ()  [unwired: 2 in, 2 out]
        n33 = property on="Previous" class="Bool"("Visible"=w65) -> ()  [unwired: 2 in, 2 out]
        n34 = property on="Next" class="Bool"("Visible"=w65) -> ()  [unwired: 2 in, 2 out]
        n35 = property on="Code" class="Str"("Visible"=w65) -> ()  [unwired: 2 in, 2 out]
        n36 = local write "PropertyMethodType"(GDSAPI_PropertyMethodType."PropertyMethod" ("PropertyMethodType")) -> ()
        n37 = Read from Text File(file (use dialog)=w62) -> (text=w64:string, error out=w63:errorcluster)  [unwired: 3 in, 2 out]
        n38 = local write "Top Folder for all classes"(w73) -> ()
        n39 = local write "Path"(w73) -> ()
        n40 = call "BaseProvider_ConfigurationMemory.vi"("Filter_Icons"=TRUE, "Action"=enum16{"Read", "Load", "Save", "Set"}."Read") -> ("PatternOut"=w59:T16)  [unwired: 11 in, 6 out]
        n41 = local write "Code"(w66) -> ()
        n42 = Bundle By Name(cluster=w78, "Counter"=0) -> (w80:T20)
        n43 = case shown="No Error" w63 {
          tunnel: w64 -> [w84 _]
          frame No Error {
            n44 = String To Path(string=w84) -> (path=w83:path)
            n45 = property on="Top Folder for all classes" class="Path"("StartPath"=w83) -> ()  [unwired: 2 in, 2 out]
          }
          frame Error {
          }
        }
        n46 = local write "VI/Method Pattern type"(w59) -> ()
        n47 = property on="Next" class="Bool"("Strings [4]"=string[] ["Next>>"]) -> ()  [unwired: 2 in, 2 out]
        n48 = local write "ExistingClasses"(w73) -> ()
        n49 = local write "BetterNames"(TRUE ("Betternames")) -> ()
        "ProgressText" <- w66
      }
      frame "Update" {
        n50 = Unbundle By Name(w109) -> ("Files"=w101:path[])
        n51 = Empty Array?(array=w101) -> (empty?=w94:bool)
        n52 = case shown="True" w94 {
          tunnel: [_ w130] -> w107
          frame False {
          }
          frame True {
            n53 = invoke class="App" method="Clipboard.Read"() -> ("Read Clipbrd"=w135:string)  [unwired: 3 in, 2 out]
            n54 = Match Pattern(string=w135, regular expression="class") -> (offset past match=w133:i32)  [unwired: 1 in, 3 out]
            n55 = Greater Or Equal To 0?(x=w133) -> (x >= 0?=w132:bool)
            n56 = Select(t=T22."Enabled" ("Disabled"), s=w132, f=T22."Disabled and Grayed Out" ("Disabled")) -> (s? t:f=w130:T22)
          }
        }
        n57 = local read "FileList"() -> (w106:i32[])
        n58 = Not(x=w94) -> (.not. x?=w90:bool)
        "FileListText" <- w90
        n59 = for {
          tunnel: w101 -> [w128] mode=indexing
          tunnel: [w127] -> w100 mode=indexing
          n60 = Strip Path(path=w128) -> (name=w127:string)  [unwired: 1 out]
        }
        n61 = Empty Array?(array=w106) -> (empty?=w104:bool)
        n62 = case shown="False" w94 {
          tunnel: [w125 w126] -> w99
          frame False {
            w125 = "" ("Code")
            n63 = local write "Code"(w125) -> ()
          }
          frame True {
            n64 = local read "Code"() -> (w126:string)
          }
        }
        n65 = Select(t=T22."Disabled and Grayed Out" ("Disabled"), s=w104, f=T22."Enabled" ("Disabled")) -> (s? t:f=w102:T22)
        n66 = property on="FileList" class="LstBox (strict)"("Item Names"=w100) -> ()  [unwired: 2 in, 2 out]
        n67 = property on="Code" class="Str"("Visible"=w94) -> ()  [unwired: 2 in, 2 out]
        n68 = property on="RemoveSelectedFiles" class="Bool"("Visible"=w90, "DisabledEnum"=w102) -> ()  [unwired: 2 in, 2 out]
        n69 = property on="ClearList" class="Bool"("Visible"=w90) -> ()  [unwired: 2 in, 2 out]
        n70 = property on="FileList" class="LstBox (strict)"("Visible"=w90) -> ()  [unwired: 2 in, 2 out]
        n71 = local read "Tab"() -> (w92:T13)
        n72 = property on="CopyfromClipboard" class="Bool"("Visible"=w94, "DisabledEnum"=w107) -> ()  [unwired: 2 in, 2 out]
        n73 = case shown="\"Overview\"" w92 {
          tunnel: [T22."Disabled and Grayed Out" ("Disabled") T22."Enabled" ("Disabled") T22."Enabled" ("Disabled")] -> w91
          tunnel: [TRUE ("directory") w114 TRUE ("directory")] -> w88
          tunnel: [string[] ["Next>>"] ("Strings [4]") string[] ["Create classes"] ("Strings [4]") string[] ["Next>>"] ("Strings [4]")] -> w87
          frame "Select" {
          }
          frame "Overview" {
            n74 = local read "Top Folder for all classes"() -> (w119:path)
            n75 = Empty String/Path?(string/path=w119) -> (empty?=w115:bool)
            n76 = File/Directory Info(path=w119) -> (directory=w117:bool)  [unwired: 1 in, 6 out]
            n77 = Not(x=w115) -> (.not. x?=w114:bool)
            n78 = Not(x=w117) -> (.not. x?=w116:bool)
            n79 = property on="Top Folder for all classes" class="Path"("Caption.Visible"=w116) -> ()  [unwired: 2 in, 2 out]
          }
          frame Default {
          }
        }
        n80 = Empty String/Path?(string/path=w99) -> (empty?=w93:bool)
        n81 = And(x=w93, y=w94) -> (x .and. y?=w96:bool)
        n82 = case shown="False" w93 {
          frame False {
            n83 = local write "Path"(path "" ("Path")) -> ()
          }
          frame True {
          }
        }
        n84 = Compound Arithmetic op=AND(invert w96, w88) -> (w89:bool)
        n85 = Select(t=T22."Enabled" ("Disabled"), s=w89, f=T22."Disabled and Grayed Out" ("Disabled")) -> (s? t:f=w95:T22)
        n86 = property on="Next" class="Bool"("DisabledEnum"=w95) -> ()  [unwired: 2 in, 2 out]
        n87 = property on="Previous" class="Bool"("DisabledEnum"=w91) -> ()  [unwired: 2 in, 2 out]
        n88 = property on="Next" class="Bool"("Strings [4]"=w87) -> ()  [unwired: 2 in, 2 out]
      }
      frame "", "Idle" {
        n89 = event shown="[18] \"Ring\": Value Change" {
          selector: _ -> [_ _ _ _ _ _ _ _ _ _ _ _ _ _ _ _ _ _ _ _]
          dyn-events: _ -> [_ _ _ _ _ _ _ _ _ _ _ _ _ _ _ _ _ _ _ _]
          timeout: 250 -> [_ _ _ _ _ _ _ _ _ _ _ _ _ _ _ _ _ _ _ _]
          tunnel: w144 -> [w147 w150 w153 w158 w195 w201 w214 w235 w237 w290 w297 w299 w307 w329 w335 w341 w343 w345 w349 w356]
          tunnel: [w147 w150 w152 w157 w195 w202 w215 w235 w236 w290 w297 w299 w305 w329 w335 w336 w343 w345 w348 w355] -> w143
          tunnel: [w145 "Update" "Exit" "CheckFiles" "Update" "Update" "Update" "Update" w239 "Update" _ "Summary" "Missing:Init" w328 "Exit" "Update" "Missing:CheckScrollPos" "Missing:HideRing" "Missing:Redraw" w354] -> w142
          tunnel: w140 -> [_ _ _ w155 _ _ _ _ _ _ _ _ _ _ _ _ _ _ _ _]
          tunnel: w139 -> [_ _ _ _ _ _ w210 _ _ _ _ _ _ _ _ _ _ _ _ _]
          tunnel: w138 -> [_ _ _ _ _ _ _ _ _ _ w294 _ _ _ _ _ _ _ _ _]
          tunnel: w137 -> [_ _ _ _ _ _ _ _ _ w288 _ _ _ _ _ _ _ _ _ _]
          event Timeout {
            n90 = event-data() -> ()  [unwired: 1 in, 2 out]
            n91 = local read "Tab"() -> (w146:T13)
            n92 = case shown="Default" w146 {
              tunnel: ["Update" _] -> w145
              frame "Select" {
              }
              frame Default {
              }
            }
          }
          event "Code": Value Change {
            n93 = event-data() -> ()  [unwired: 1 in, 5 out]
          }
          event Panel Close? {
            w151 = TRUE ("Discard?")
            n94 = event-data() -> ()  [unwired: 1 in, 1 out]
            n95 = Bundle By Name(cluster=w153, "Cancelled"=w151) -> (w152:T20)
            n96 = event-data("Discard?"=w151) -> ()  [unwired: 1 in, 1 out]
          }
          event "Path": Value Change {
            n97 = event-data() -> ()  [unwired: 1 in, 3 out]
            n98 = Empty String/Path?(string/path="Path") -> (empty?=w159:bool)
            n99 = case shown="False" w159 {
              tunnel: "Path" -> [w167 _]
              tunnel: w158 -> [w165 w193]
              tunnel: [w163 w193] -> w157
              tunnel: w155 -> [w161 _]
              frame False {
                n100 = File/Directory Info(path=w167) -> (path out=w164:path, directory=w166:bool, error out=w162:errorcluster)  [unwired: 1 in, 4 out]
                n101 = case shown="No Error" w162 {
                  tunnel: w166 -> [w174 _]
                  tunnel: w165 -> [w173 w192]
                  tunnel: w164 -> [w172 _]
                  tunnel: [w171 w192] -> w163
                  tunnel: w161 -> [w168 _]
                  frame No Error {
                    n102 = case shown="True" w174 {
                      tunnel: w173 -> [w180 w190]
                      tunnel: w172 -> [w183 w187]
                      tunnel: [w181 w191] -> w171
                      tunnel: [w175 w186] -> w169
                      frame True {
                        n103 = Unbundle By Name(w180) -> ("Files"=w179:path[])
                        n104 = call <vilib>:"Recursive File List.vi"("pattern"="*.cs", "Folder Path"=w183) -> ("All Files in Dir"=w177:path[], "dup Folder Path"=w182:path)  [unwired: 5 in, 3 out]
                        n105 = call <vilib>:"Recursive File List.vi"("pattern"="*.java", "Folder Path"=w182) -> ("All Files in Dir"=w176:path[], "dup Folder Path"=w175:path)  [unwired: 5 in, 3 out]
                        n106 = Build Array (concatenate)(w179, w177, w176) -> (w178:path[])
                        n107 = Bundle By Name(cluster=w180, "Files"=w178) -> (w181:T20)
                      }
                      frame False {
                        n108 = Unbundle By Name(w190) -> ("Files"=w189:path[])
                        n109 = Build Array (concatenate)(w189, w187) -> (w188:path[])
                        n110 = Strip Path(path=w187) -> (stripped path=w186:path)  [unwired: 1 out]
                        n111 = Bundle By Name(cluster=w190, "Files"=w188) -> (w191:T20)
                      }
                    }
                    n112 = Path To String(path=w169) -> (string=w170:string)
                    n113 = Write to Text File(file (use dialog)=w168, text=w170) -> ()  [unwired: 2 in, 3 out]
                  }
                  frame Error {
                  }
                }
              }
              frame True {
              }
            }
          }
          event "FileList": Value Change {
            n114 = event-data() -> ()  [unwired: 1 in, 3 out]
          }
          event "RemoveSelectedFiles": Value Change {
            n115 = event-data() -> ()  [unwired: 1 in, 3 out]
            n116 = local read "FileList"() -> (w199:i32[])
            n117 = Reverse 1D Array(array=w199) -> (reversed array=w197:i32[])
            n118 = Unbundle By Name(w201) -> ("Files"=w200:path[])
            n119 = for {
              shift-right: [w208] -> w198
              shift-left: w200 -> [w209]
              tunnel: w197 -> [w207] mode=indexing
              n120 = Delete From Array(array=w209, index=w207) -> (array with subset deleted=w208:path[])  [unwired: 1 in, 1 out]
            }
            n121 = stacked-sequence {
              tunnel: [w206] -> w202
              tunnel: w201 -> [w205]
              tunnel: w198 -> [w204]
              frame #0 {
                n122 = Bundle By Name(cluster=w205, "Files"=w204) -> (w206:T20)
                n123 = local write "FileList"(i32[] [] ("FileList")) -> ()
              }
            }
          }
          event "FileList": Double Click {
            n124 = event-data() -> ("Row"=w212:i32, "PlatMods.Ctrl"=w211:bool)  [unwired: 1 in]
            n125 = case shown="True" w211 {
              tunnel: [w220 w231] -> w215
              tunnel: w214 -> [w219 w231]
              tunnel: w212 -> [w216 w230]
              tunnel: w210 -> [_ w225]
              frame False {
                n126 = Unbundle By Name(w219) -> ("Files"=w218:path[])
                n127 = Delete From Array(array=w218, index=w216) -> (array with subset deleted=w217:path[])  [unwired: 1 in, 1 out]
                n128 = stacked-sequence {
                  tunnel: [w224] -> w220
                  tunnel: w219 -> [w223]
                  tunnel: w217 -> [w222]
                  frame #0 {
                    n129 = Bundle By Name(cluster=w223, "Files"=w222) -> (w224:T20)
                    n130 = local write "FileList"(i32[] [] ("FileList")) -> ()
                  }
                }
              }
              frame True {
                n131 = Unbundle By Name(w231) -> ("Files"=w232:path[])
                n132 = Index Array(array=w232, index=w230) -> (element=w229:path)
                n133 = Format Into String(format string=" \"%s\"", initial string=w225, w229) -> (resulting string=w226:string)  [unwired: 1 in, 1 out]
                n134 = call <vilib>:"System Exec.vi"("wait until completion? (T)"=FALSE, "command line"=w226) -> ()  [unwired: 6 in, 4 out]
              }
            }
          }
          event "CopyfromClipboard": Value Change {
            n135 = event-data() -> ()  [unwired: 1 in, 3 out]
            n136 = invoke class="App" method="Clipboard.Read"() -> ("Read Clipbrd"=w234:string)  [unwired: 3 in, 2 out]
            n137 = local write "Code"(w234) -> ()
          }
          event "Next": Value Change {
            n138 = event-data() -> ()  [unwired: 1 in, 3 out]
            n139 = local read "Tab"() -> (w238:T13)
            n140 = case shown="\"Missing\"" w238 {
              tunnel: ["AnalyseFiles" w250 "Idle" "CreateClasses"] -> w239
              tunnel: w237 -> [_ w249 _ _]
              tunnel: w237 -> [w240 w245 w268 w270]
              tunnel: [w240 w244 w268 w270] -> w236
              frame "Select" {
              }
              frame "Missing" {
                n141 = Unbundle By Name(w249) -> ("Interface"=w242:bool, "InterfaceItems"=w248:T18[], "MissingTypes.Selected"=w243:i32[])
                n142 = Empty Array?(array=w248) -> (empty?=w247:bool)
                n143 = Or(x=w242, y=w247) -> (x .or. y?=w246:bool)
                n144 = case shown="True" w246 {
                  tunnel: ["Missing:Start" "Update"] -> w250
                  tunnel: w245 -> [w254 w259]
                  tunnel: [w253 w258] -> w244
                  tunnel: w243 -> [w251 w256]
                  tunnel: w242 -> [_ w257]
                  frame False {
                    n145 = Bundle By Name(cluster=w254, "Interface"=TRUE, "MissingTypeSelected"=w251) -> (w253:T20)
                  }
                  frame True {
                    n146 = case shown="True" w257 {
                      tunnel: w259 -> [w264 w267]
                      tunnel: [w263 w266] -> w258
                      tunnel: w256 -> [w262 w265]
                      frame True {
                        n147 = Bundle By Name(cluster=w264, "InterfaceSelected"=w262) -> (w263:T20)
                      }
                      frame False {
                        n148 = Bundle By Name(cluster=w267, "MissingTypeSelected"=w265) -> (w266:T20)
                      }
                    }
                    n149 = property on="Tab" class="TabCtl (strict)"("Value"=T13."Overview" ("Tab")) -> ()  [unwired: 2 in, 2 out]
                  }
                }
              }
              frame Default {
              }
              frame "Overview" {
                n150 = local read "Top Folder for all classes"() -> (w271:path)
                n151 = List Folder(path=w271) -> (filenames=w274:string[], folder names=w275:string[])  [unwired: 3 in, 2 out]
                n152 = Empty Array?(array=w275) -> (empty?=w276:bool)
                n153 = Empty Array?(array=w274) -> (empty?=w273:bool)
                n154 = And(x=w273, y=w276) -> (x .and. y?=w272:bool)
                n155 = case shown="True" w272 {
                  tunnel: w271 -> [w278 _]
                  frame False {
                    n156 = Two Button Dialog(message="Top Folder not empty", 1:"Continue" ("F button name (\"Cancel\")"), 2:"Empty folder now" ("T button name (\"OK\")")) -> (T button?=w279:bool)
                    n157 = case shown="True" w279 {
                      tunnel: w278 -> [_ w284]
                      frame False {
                      }
                      frame True {
                        n158 = call <vilib>:"Recursive File List.vi"("Folder Path"=w284) -> ("All Files in Dir"=w283:path[])  [unwired: 6 in, 4 out]
                        n159 = for {
                          tunnel: w283 -> [w285] mode=indexing
                          n160 = Delete(path (use dialog)=w285) -> ()  [unwired: 4 in, 3 out]
                        }
                      }
                    }
                  }
                  frame True {
                  }
                }
              }
            }
          }
          event "Top Folder for all classes": Value Change {
            n161 = event-data() -> ()  [unwired: 1 in, 3 out]
            n162 = Empty String/Path?(string/path="Top Folder for all classes") -> (empty?=w286:bool)
            n163 = case shown="False" w286 {
              tunnel: w288 -> [w292 _]
              tunnel: "Top Folder for all classes" -> [w291 _]
              frame False {
                n164 = Path To String(path=w291) -> (string=w293:string)
                n165 = Write to Text File(file (use dialog)=w292, text=w293) -> ()  [unwired: 2 in, 3 out]
              }
              frame True {
              }
            }
          }
          event "ClassType": Value Change {
            n166 = event-data() -> ()  [unwired: 1 in, 3 out]
            n167 = Format Into String("ClassType") -> (resulting string=w295:string)  [unwired: 3 in, 1 out]
            n168 = Write to Text File(file (use dialog)=w294, text=w295) -> ()  [unwired: 2 in, 3 out]
          }
          event "ViewClassOverView": Value Change {
            n169 = event-data() -> ()  [unwired: 1 in, 3 out]
          }
          event "ExistingClasses": Value Change {
            n170 = event-data() -> ()  [unwired: 1 in, 3 out]
            n171 = Unbundle By Name(w307) -> ("ExistingClassesFolders"=w302:path[], "MissingItems"=w306:T18[])
            n172 = call <vilib>:"Recursive File List.vi"("pattern"="*.lvclass", "Folder Path"="ExistingClasses") -> ("All Files in Dir"=w313:path[])  [unwired: 5 in, 4 out]
            n173 = call <vilib>:"Recursive File List.vi"("pattern"="*.ctl", "Folder Path"="ExistingClasses") -> ("All Files in Dir"=w312:path[])  [unwired: 5 in, 4 out]
            n174 = for {
              tunnel: w313 -> [w325] mode=indexing
              tunnel: [w324] -> w311 mode=indexing
              n175 = call <vilib>:"Get File Extension.vi"("file"=w325) -> ("filename without extension"=w324:string)  [unwired: 6 in, 4 out]
            }
            n176 = for {
              tunnel: w312 -> [w323] mode=indexing
              tunnel: [w322] -> w310 mode=indexing
              n177 = call <vilib>:"Get File Extension.vi"("file"=w323) -> ("filename without extension"=w322:string)  [unwired: 6 in, 4 out]
            }
            n178 = Build Array (concatenate)(w311, w310) -> (w309:string[])
            n179 = To Lower Case(string=w309) -> (all lower case string=w308:string[])
            n180 = for {
              tunnel: w308 -> [w321]
              tunnel: [w316] -> w304 mode=indexing if=w319
              tunnel: w306 -> [w316] mode=indexing
              n181 = Unbundle By Name(w316) -> ("Item"=w317:string)
              n182 = To Lower Case(string=w317) -> (all lower case string=w318:string)
              n183 = Search 1D Array(1D array=w321, element=w318) -> (index of element=w320:i32)  [unwired: 1 in]
              n184 = Less Than 0?(x=w320) -> (x < 0?=w319:bool)
            }
            n185 = Build Array (concatenate)(w302, "ExistingClasses") -> (w300:path[])
            n186 = Bundle By Name(cluster=w307, "ExistingClassesFolders"=w300, "MissingItems"=w304) -> (w305:T20)
          }
          event "Previous": Value Change {
            n187 = event-data() -> ()  [unwired: 1 in, 3 out]
            n188 = local read "Tab"() -> (w327:T13)
            n189 = case shown="\"Select\"" w327 {
              tunnel: ["AnalyseFiles" "Update" "Idle"] -> w328
              frame "Select" {
              }
              frame "Missing", "Overview" {
                n190 = property on="Tab" class="TabCtl (strict)"("Value"=T23."Select" ("Tab")) -> ()  [unwired: 2 in, 2 out]
              }
              frame Default {
              }
            }
            n191 = property on="Next" class="Bool"("Strings [4]"=string[] ["Next>>"]) -> ()  [unwired: 2 in, 2 out]
          }
          event "Cancel": Value Change {
            n192 = event-data() -> ()  [unwired: 1 in, 3 out]
          }
          event "ClearList": Value Change {
            n193 = event-data() -> ()  [unwired: 1 in, 3 out]
            n194 = local write "FileList"(i32[] [] ("FileList")) -> ()
            n195 = local write "Path"(path "" ("Path")) -> ()
            n196 = Bundle By Name(cluster=w341, "Files"=path[] []) -> (w336:T20)
          }
          event "Picture": Mouse Down; "Picture": Mouse Up; "Picture": Mouse Leave {
            n197 = event-data() -> ()  [unwired: 1 in, 1 out]
          }
          event "Ring": Mouse Leave {
            n198 = event-data() -> ()  [unwired: 1 in, 1 out]
          }
          event "Ring": Value Change {
            n199 = event-data() -> ()  [unwired: 1 in, 3 out]
            n200 = Unbundle By Name(w349) -> ("MissingTypes.Selected"=w352:i32[], "MissingTypes.Row"=w351:i32)
            n201 = in-place {
              in-place-border: "Ring" -> [w353]
              n202 = in-place-array #1(w352, w351) -> ()  [unwired: 1 out]
              n203 = in-place-array #1(w353) -> (w350:i32[])  [unwired: 1 out]
            }
            n204 = Bundle By Name(cluster=w349, "MissingTypes.Selected"=w350) -> (w348:T20)
          }
          event "Picture": Mouse Move {
            n205 = event-data() -> ()  [unwired: 1 in, 2 out]
            n206 = Unbundle By Name(w356) -> ("MissingTypes.ShowRing"=w365:bool)
            n207 = property on="Picture" class="Pict"() -> ("Mouse"=w367:T29)  [unwired: 2 in, 2 out]
            n208 = Unbundle By Name(w367) -> ("Mouse Position"=w366:cluster{"X":i32, "Y":i32})
            n209 = Unbundle By Name(w356) -> ("MissingTypes.IndexOffset"=w363:i32, "MissingTypes.VerticalRows"=w357:i32, "MissingTypes.Rectangles"=w358:T30)
            n210 = for {
              tunnel: w358 -> [w378] mode=indexing
              tunnel: w366 -> [w380]
              tunnel: [w379] -> w368
              tunnel: [w378] -> w364
              tunnel: [w377] -> w361
              i -> [w377]
              stop <- w379 stop-if-true
              n211 = call <vilib>:"PointInRect.vi"("rect"=w378, "point"=w380) -> ("pt in rect"=w379:bool)
            }
            n212 = Add(x=w363, y=w357) -> (x+y=w362:i32)
            n213 = Decrement(x=w362) -> (x-1=w360:i32)
            n214 = Less Or Equal?(x=w361, y=w360) -> (x <= y?=w359:bool)
            n215 = Compound Arithmetic op=AND(w359, w368, invert w365) -> (w369:bool)
            n216 = case shown="True" w369 {
              tunnel: w364 -> [_ _]
              tunnel: w368 -> [w373 _]
              tunnel: w365 -> [w371 _]
              tunnel: [w370 "Missing:ShowRing"] -> w354
              frame False {
                n217 = Compound Arithmetic op=AND(invert w373, w371) -> (w372:bool)
                n218 = case shown="True" w372 {
                  tunnel: ["Idle" ("format string") "Missing:HideRing"] -> w370
                  frame False {
                  }
                  frame True {
                  }
                }
              }
              frame True {
              }
            }
            n219 = Bundle By Name(cluster=w356, "MissingTypes.Row"=w361, "MissingTypes.Rectangle"=w364) -> (w355:T20)
          }
        }
      }
      frame "AnalyseFiles" {
        w388 = T23."Analysing" ("Tab")
        n220 = local read "Code"() -> (w396:string)
        n221 = Unbundle By Name(w397) -> ("Files"=w394:path[])
        n222 = call <vilib>:"Trim Whitespace.vi"("string"=w396) -> ("trimmed string"=w395:string)  [unwired: 1 in]
        n223 = case shown="Default" w395 {
          selector: w395 -> [w425 _]
          tunnel: w394 -> [_ w428]
          tunnel: [w423 w428] -> w393
          tunnel: w388 -> [_ _]
          frame Default {
            n224 = Temporary Directory() -> (w426:path)
            n225 = Build Path(base path=w426, name or relative path="GDS_CodeTempFile.txt") -> (appended path=w424:path)
            n226 = Write to Text File(file (use dialog)=w424, text=w425) -> ()  [unwired: 2 in, 3 out]
            n227 = Build Array(w424) -> (w423:path[])
          }
          frame "" {
          }
        }
        n228 = call <vilib>:"Set Busy.vi"("error in (no error)"=w399) -> ("error out"=w390:errorcluster)  [unwired: 9 in, 1 out]
        n229 = property on="Tab" class="TabCtl (strict)"("Value"=w388) -> ()  [unwired: 2 in, 2 out]
        n230 = for {
          shift-right: [w422] -> w398
          shift-left: w390 -> [w419]
          tunnel: w393 -> [w420] mode=indexing
          tunnel: [w417] -> w387 mode=concatenating
          tunnel: [w416] -> w386 mode=concatenating
          tunnel: [w415] -> w385 mode=concatenating
          n231 = Read from Text File(file (use dialog)=w420, error in=w419) -> (text=w421:string, error out=w418:errorcluster)  [unwired: 2 in, 2 out]
          n232 = call "GDSString_ParseTextBasedCode.vi"("error in (no error)"=w418, "TextIn"=w421) -> ("error out"=w422:errorcluster, "EnumsOusideClass"=w415:T11[], "StructsOusideClass"=w416:T12[], "Classes"=w417:T1[])  [unwired: 6 in]
        }
        n233 = for {
          N: 10 -> [_]
          shift-right: [w402] -> w384
          shift-left: w387 -> [w410]
          shift-right: [w401] -> w383
          shift-left: w386 -> [w409]
          shift-right: [w403] -> w382
          shift-left: w385 -> [w408]
          stop <- w400 stop-if-true
          n234 = call "ConvertTextBasedCodeToLabVIEW_CreateMissingTypeList.vi"("EnumsOusideClass"=w408, "StructsOusideClass"=w409, "Classes"=w410) -> ("MissingItems"=w407:T18[])  [unwired: 8 in]
          n235 = call "ConvertTextBasedCodeToLabVIEW_CreateCommonItems.vi"("MissingItems"=w407) -> ("EnumsOusideClass"=w404:T11[], "StructsOusideClass"=w405:T12[], "Classes"=w406:T1[], "NothingAdded"=w400:bool)  [unwired: 6 in, 1 out]
          n236 = Build Array (concatenate)(w410, w406) -> (w402:T1[])
          n237 = Build Array (concatenate)(w409, w405) -> (w401:T12[])
          n238 = Build Array (concatenate)(w408, w404) -> (w403:T11[])
        }
        "Classes" <- w384
        n239 = Bundle By Name(cluster=w397, "Classes"=w384, "StructsOusideClass"=w383, "EnumsOusideClass"=w382) -> (w392:T20)
        n240 = Empty Array?(array=w384) -> (empty?=w389:bool)
        n241 = case shown="False" w389 {
          tunnel: ["UpdateClassParentType" "Update"] -> w391
          frame False {
          }
          frame True {
            n242 = property on="Tab" class="TabCtl (strict)"("Value"=T23."Select" ("Tab")) -> ()  [unwired: 2 in, 2 out]
            n243 = One Button Dialog(message="No classes found") -> ()  [unwired: 1 in, 1 out]
            n244 = call <vilib>:"Unset Busy.vi"() -> ()  [unwired: 11 in, 1 out]
          }
        }
      }
      frame "UpdateClassParentType" {
        n245 = Unbundle By Name(w432) -> ("Classes"=w435:T1[])
        n246 = for {
          tunnel: w435 -> [w458] mode=indexing
          tunnel: [w457] -> w434 mode=indexing
          tunnel: [w456] -> w433 mode=indexing
          n247 = Unbundle By Name(w458) -> ("ClassName"=w457:string, "ClassType"=w456:T9)
        }
        n248 = for {
          tunnel: w435 -> [w439] mode=indexing
          tunnel: w434 -> [w441]
          tunnel: w433 -> [w440]
          tunnel: [w437] -> w430 mode=indexing
          n249 = Unbundle By Name(w439) -> ("ParentClasses"=w442:T8[])
          n250 = for {
            tunnel: w442 -> [w445] mode=indexing
            tunnel: w441 -> [w447]
            tunnel: w440 -> [w446]
            tunnel: [w443] -> w438 mode=indexing
            n251 = Unbundle By Name(w445) -> ("ClassName"=w448:string, "ClassType"=w449:T9)
            n252 = case shown="\"Undefined\"" w449 {
              selector: w449 -> [w450 _]
              tunnel: w448 -> [_ w455]
              tunnel: w447 -> [_ w454]
              tunnel: w446 -> [_ w453]
              tunnel: [w450 w451] -> w444
              frame Default {
              }
              frame "Undefined" {
                n253 = Search 1D Array(1D array=w454, element=w455) -> (index of element=w452:i32)  [unwired: 1 in]
                n254 = Index Array(array=w453, index=w452) -> (element=w451:T9)
              }
            }
            n255 = Bundle By Name(cluster=w445, "ClassType"=w444) -> (w443:T8)
          }
          n256 = Bundle By Name(cluster=w439, "ParentClasses"=w438) -> (w437:T1)
        }
        n257 = Bundle By Name(cluster=w432, "Classes"=w430) -> (w431:T20)
      }
      frame "ReplaceDataTypeOther" {
        # "List of all types (classes,Interfaces,Enums,structs)"
        n258 = Unbundle By Name(w466) -> ("Classes"=w468:T1[], "StructsOusideClass"=w460:T12[], "EnumsOusideClass"=w459:T11[])
        n259 = call "ConvertTextBasedCodeToLabVIEW_GetDataTypeNames.vi"("EnumsOusideClass"=w459, "StructsOusideClass"=w460, "Classes"=w468) -> ("DataType:Name"=w467:string[], "DataType:Type"=w463:T6[])  [unwired: 7 in]
        n260 = for {
          tunnel: w468 -> [w477] mode=indexing
          tunnel: w467 -> [w470]
          tunnel: w463 -> [w469]
          tunnel: [w475] -> w461 mode=indexing
          n261 = Unbundle By Name(w477) -> ("Attributes"=w478:T5[], "Structs"=w474:T12[], "Methods"=w472:T4[])
          n262 = for {
            tunnel: w474 -> [w521] mode=indexing
            tunnel: w470 -> [w523]
            tunnel: w469 -> [w522]
            tunnel: [w519] -> w473 mode=indexing
            n263 = Unbundle By Name(w521) -> ("Items"=w524:T5[])
            n264 = for {
              tunnel: w524 -> [w529] mode=indexing
              tunnel: w523 -> [w531]
              tunnel: w522 -> [w530]
              tunnel: [w527] -> w520 mode=indexing
              n265 = Unbundle By Name(w529) -> ("DataType"=w526:T6, "DataTypeString"=w525:string)
              n266 = case shown="\"LabVIEW Class\", \"TypeDef\", \"Other\"" w526 {
                selector: w526 -> [w532 w533]
                tunnel: w525 -> [_ w538]
                tunnel: w531 -> [_ w537]
                tunnel: w530 -> [_ w536]
                tunnel: [w532 w535] -> w528
                frame Default {
                }
                frame "LabVIEW Class", "TypeDef", "Other" {
                  n267 = Search 1D Array(1D array=w537, element=w538) -> (index of element=w534:i32)  [unwired: 1 in]
                  n268 = case shown="Default" w534 {
                    selector: w534 -> [w539 _]
                    tunnel: w536 -> [w541 _]
                    tunnel: [w540 w542] -> w535
                    tunnel: w533 -> [_ w542]
                    frame Default {
                      n269 = Index Array(array=w541, index=w539) -> (element=w540:T6)
                    }
                    frame -1 {
                    }
                  }
                }
              }
              n270 = Bundle By Name(cluster=w529, "DataType"=w528) -> (w527:T5)
            }
            n271 = Bundle By Name(cluster=w521, "Items"=w520) -> (w519:T12)
          }
          n272 = for {
            tunnel: w472 -> [w488] mode=indexing
            tunnel: [w486] -> w471 mode=indexing
            tunnel: w470 -> [w481]
            tunnel: w469 -> [w480]
            n273 = Unbundle By Name(w488) -> ("MethodArguments"=w489:T5[], "ReturnType"=w483:T5)
            n274 = for {
              tunnel: w489 -> [w505] mode=indexing
              tunnel: w481 -> [w507]
              tunnel: w480 -> [w506]
              tunnel: [w503] -> w487 mode=indexing
              n275 = Unbundle By Name(w505) -> ("DataType"=w502:T6, "DataTypeString"=w501:string)
              n276 = case shown="\"LabVIEW Class\", \"TypeDef\", \"Other\"" w502 {
                selector: w502 -> [w508 w509]
                tunnel: w501 -> [_ w514]
                tunnel: w507 -> [_ w513]
                tunnel: w506 -> [_ w512]
                tunnel: [w508 w511] -> w504
                frame Default {
                }
                frame "LabVIEW Class", "TypeDef", "Other" {
                  n277 = Search 1D Array(1D array=w513, element=w514) -> (index of element=w510:i32)  [unwired: 1 in]
                  n278 = case shown="Default" w510 {
                    selector: w510 -> [w515 _]
                    tunnel: w512 -> [w517 _]
                    tunnel: [w516 w518] -> w511
                    tunnel: w509 -> [_ w518]
                    frame Default {
                      n279 = Index Array(array=w517, index=w515) -> (element=w516:T6)
                    }
                    frame -1 {
                    }
                  }
                }
              }
              n280 = Bundle By Name(cluster=w505, "DataType"=w504) -> (w503:T5)
            }
            n281 = Unbundle By Name(w483) -> ("DataType"=w484:T6, "DataTypeString"=w485:string)
            n282 = case shown="\"LabVIEW Class\", \"TypeDef\", \"Other\"" w484 {
              selector: w484 -> [w490 w491]
              tunnel: w485 -> [_ w496]
              tunnel: w481 -> [_ w495]
              tunnel: w480 -> [_ w494]
              tunnel: [w490 w493] -> w479
              frame Default {
              }
              frame "LabVIEW Class", "TypeDef", "Other" {
                n283 = Search 1D Array(1D array=w495, element=w496) -> (index of element=w492:i32)  [unwired: 1 in]
                n284 = case shown="Default" w492 {
                  selector: w492 -> [w497 _]
                  tunnel: w494 -> [w499 _]
                  tunnel: [w498 w500] -> w493
                  tunnel: w491 -> [_ w500]
                  frame Default {
                    n285 = Index Array(array=w499, index=w497) -> (element=w498:T6)
                  }
                  frame -1 {
                  }
                }
              }
            }
            n286 = Bundle By Name(cluster=w483, "DataType"=w479) -> (w482:T5)
            n287 = Bundle By Name(cluster=w488, "MethodArguments"=w487, "ReturnType"=w482) -> (w486:T4)
          }
          n288 = for {
            tunnel: w478 -> [w547] mode=indexing
            tunnel: w470 -> [w549]
            tunnel: w469 -> [w548]
            tunnel: [w545] -> w476 mode=indexing
            n289 = Unbundle By Name(w547) -> ("DataType"=w544:T6, "DataTypeString"=w543:string)
            n290 = case shown="\"LabVIEW Class\", \"TypeDef\", \"Other\"" w544 {
              selector: w544 -> [w550 w551]
              tunnel: w543 -> [_ w556]
              tunnel: w549 -> [_ w555]
              tunnel: w548 -> [_ w554]
              tunnel: [w550 w553] -> w546
              frame Default {
              }
              frame "LabVIEW Class", "TypeDef", "Other" {
                n291 = Search 1D Array(1D array=w555, element=w556) -> (index of element=w552:i32)  [unwired: 1 in]
                n292 = case shown="Default" w552 {
                  selector: w552 -> [w557 _]
                  tunnel: w554 -> [w559 _]
                  tunnel: [w558 w560] -> w553
                  tunnel: w551 -> [_ w560]
                  frame Default {
                    n293 = Index Array(array=w559, index=w557) -> (element=w558:T6)
                  }
                  frame -1 {
                  }
                }
              }
            }
            n294 = Bundle By Name(cluster=w547, "DataType"=w546) -> (w545:T5)
          }
          n295 = Bundle By Name(cluster=w477, "Attributes"=w476, "Structs"=w473, "Methods"=w471) -> (w475:T1)
        }
        n296 = local write "Classes"(w461) -> ()
        n297 = Bundle By Name(cluster=w466, "Classes"=w461) -> (w465:T20)
      }
      frame "FindGenericTypes" {
        n298 = Unbundle By Name(w564) -> ("Classes"=w565:T1[])
        n299 = call "ConvertTextBasedCodeToLabVIEW_FindGenerics.vi"("Classes"=w565) -> ("ClassesOut"=w562:T1[])  [unwired: 10 in]
        n300 = Bundle By Name(cluster=w564, "Classes"=w562) -> (w563:T20)
      }
      frame "CheckDependencies" {
        (unwired) ConvertTextBasedCodeToLabVIEW_MissingTypeIconType."?" ("Icon")
        w571 = T18[] [] ("InterfaceItems")
        # "LV2020 Support Interface classes"
        n301 = Unbundle By Name(w570) -> ("Classes"=w573:T1[], "StructsOusideClass"=w575:T12[], "EnumsOusideClass"=w574:T11[])
        n302 = call "ConvertTextBasedCodeToLabVIEW_CreateMissingTypeList.vi"("EnumsOusideClass"=w574, "StructsOusideClass"=w575, "Classes"=w573) -> ("MissingItems"=w576:T18[])  [unwired: 8 in]
        n303 = call "ConvertTextBasedCodeToLabVIEW_CreateInterfaceList.vi"("Classes"=w573) -> ()  [unwired: 10 in, 1 out]
        n304 = Empty Array?(array=w571) -> (empty?=w567:bool)
        n305 = Empty Array?(array=w576) -> (empty?=w568:bool)
        n306 = Bundle By Name(cluster=w570, "MissingItems"=w576, "InterfaceItems"=w571, "Interface"=w568) -> (w569:T20)
        n307 = And(x=w568, y=w567) -> (x .and. y?=w572:bool)
        n308 = case shown="False" w572 {
          tunnel: ["Missing:Start" "Update"] -> w579
          tunnel: w568 -> [_ _]
          tunnel: w571 -> [_ _]
          frame False {
          }
          frame True {
            n309 = property on="Tab" class="TabCtl (strict)"("Value"=T13."Overview" ("Tab")) -> ()  [unwired: 2 in, 2 out]
          }
        }
        n310 = call <vilib>:"Unset Busy.vi"("error in (no error)"=w577) -> ("error out"=w578:errorcluster)  [unwired: 10 in]
      }
      frame "----- Missing Types ------" {
      }
      frame "Missing:Start" {
        n311 = Unbundle By Name(w589) -> ("Interface"=w588:bool)
        n312 = Not(x=w588) -> (.not. x?=w594:bool)
        n313 = property on="Previous" class="Bool"("DisabledEnum"=T22."Enabled" ("Disabled")) -> ()  [unwired: 2 in, 2 out]
        n314 = property on="Tab" class="TabCtl (strict)"("Value"=T13."Missing" ("Tab")) -> ()  [unwired: 2 in, 2 out]
        n315 = Select(t=w587, s=w594, f=w586) -> (s? t:f=w595:string)
        n316 = Select(t=w585, s=w594, f="") -> (s? t:f=w593:string)
        n317 = property on="ExistingClasses" class="Path"("Visible"=w594) -> ()  [unwired: 2 in, 2 out]
        n318 = local write "MissingText2"(w593) -> ()
        n319 = local write "MissingText1"(w595) -> ()
      }
      frame "Missing:Init" {
        w611 = 18  # Y-Distance
        n320 = Unbundle By Name(w602) -> ("InterfaceItems"=w600:T18[], "Interface"=w601:bool, "MissingItems"=w599:T18[])
        n321 = Unbundle By Name(w602) -> ("MissingTypes.XStart1"=w621:i32, "MissingTypes.HorGap"=w617:i32, "MissingTypes.VerGap"=w615:i32, "MissingTypes.UserFont"=w625:T31, "MissingTypes.Font"=w624:T32)
        n322 = Select(t=w600, s=w601, f=w599) -> (s? t:f=w598:T18[])
        n323 = for {
          tunnel: [w647] -> w608 mode=indexing
          tunnel: w624 -> [w646]
          tunnel: w625 -> [w645]
          tunnel: [w643] -> w609 mode=indexing
          tunnel: [w642] -> w610 mode=indexing
          tunnel: w598 -> [w640] mode=indexing
          n324 = Unbundle By Name(w640) -> ("Index"=w647:i32, "Item"=w641:string)  [unwired: 1 out]
          n325 = call <vilib>:"Get Text Rect.vi"("desired font(Application)"=w646, "text"=w641, "[user-specified font]"=w645) -> ("rect"=w644:T25)  [unwired: 6 in]
          n326 = Unbundle(w644) -> ("right"=w643:i16, "bottom"=w642:i16)  [unwired: 2 out]
        }
        n327 = Array Max & Min(array=w609) -> (max value=w616:i16)  [unwired: 3 out]
        n328 = Array Max & Min(array=w610) -> (max value=w612:i16)  [unwired: 3 out]
        n329 = Add(x=w617, y=w616) -> (x+y=w618:i32)
        n330 = Add(x=w615, y=w612) -> (x+y=w613:i32)
        n331 = Max & Min(x=200, y=w618) -> (min(x,y)=w620:i32)  [unwired: 1 out]
        n332 = Max & Min(x=w613, y=w611) -> (max(x,y)=w614:i32)  [unwired: 1 out]
        n333 = case shown="\"Application Font\"" w624 {
          tunnel: [T24 {"Font Name"="Dlg Font", "Size"=15, "Bold"=FALSE, "Italic"=FALSE, "Underline"=FALSE, "Strikeout"=FALSE, "Color"=16777228} ("Ring Text.Font") T24 {"Font Name"="App Font", "Size"=15, "Bold"=FALSE, "Italic"=FALSE, "Underline"=FALSE, "Strikeout"=FALSE, "Color"=16777228} ("Ring Text.Font") w638] -> w623
          tunnel: w625 -> [_ _ w637]
          frame Default {
          }
          frame "Application Font" {
          }
          frame "User-specified Font" {
            n334 = Unbundle(w637) -> ("Font Name:"=w636:string, "Size"=w635:i16, "Strikeout?"=w631:bool, "Italic?"=w633:bool, "Underline?"=w632:bool, "Bold?"=w634:bool)  [unwired: 2 out]
            n335 = Bundle(cluster=T24 {"Font Name"="", "Size"=0, "Bold"=FALSE, "Italic"=FALSE, "Underline"=FALSE, "Strikeout"=FALSE, "Color"=0} ("Ring Text.Font"), "Font Name"=w636, "Size"=w635, "Bold"=w634, "Italic"=w633, "Underline"=w632, "Strikeout"=w631, "Color"=u32 0) -> (w638:T24)
          }
        }
        n336 = Add(x=w621, y=w620) -> (x+y=w622:i32)
        n337 = Bundle By Name(cluster=w602, "MissingTypes.Selected"=w608, "MissingTypes.XStart2"=w622, "MissingTypes.Y-Distance"=w614) -> (w604:T20)
        n338 = Bundle By Name(cluster=w623, "Color"=u32 1673) -> (w626:T24)
        n339 = property on="Ring" class="Ring (strict)"("Visible"=FALSE, "RingText.Font"=w626) -> ()  [unwired: 2 in, 2 out]
        n340 = property on="Picture" class="Pict"("Top"=i16 0 ("Origin:Top")) -> ()  [unwired: 2 in, 2 out]
      }
      frame "Missing:Redraw" {
        w674 = T17 {"image type"=0, "image depth"=24, "image"=array[867 elements], "mask"=[], "colors"=[], "Rectangle"={"left"=0, "top"=0, "right"=17, "bottom"=17}}  # DropDownArrow
        n341 = Unbundle By Name(w649) -> ("InterfaceItems"=w651:T18[], "Interface"=w652:bool, "MissingItems"=w650:T18[])
        n342 = Unbundle By Name(w649) -> ("MissingTypes.Y-Distance"=w671:i32)
        n343 = property on="Picture" class="Pict"() -> ("Draw Area Size"=w665:T26)  [unwired: 2 in, 2 out]
        n344 = Select(t=w651, s=w652, f=w650) -> (s? t:f=w648:T18[])
        n345 = Unbundle By Name(w665) -> ("Width"=w664:u32, "Height"=w657:u32)
        n346 = Unbundle By Name(w649) -> ("MissingTypes.UserFont"=w668:T31, "MissingTypes.Font"=w669:T32, "MissingTypes.XStart2"=w666:i32, "MissingTypes.XStart1"=w667:i32, "MissingTypes.Selected"=w662:i32[], "MissingTypes.YStart"=w661:i32)
        n347 = Subtract(x=w664, y=u32 20) -> (x-y=w659:u32)
        n348 = for {
          N: 10 -> [_]
          shift-right: [w696] -> w655
          shift-left: picture data[5B] ("new picture") -> [w723]
          tunnel: w674 -> [w716]
          tunnel: w671 -> [w711]
          tunnel: [w709] -> w670 mode=indexing
          tunnel: w669 -> [w708]
          tunnel: w668 -> [w707]
          tunnel: w668 -> [w706]
          tunnel: w667 -> [w705]
          tunnel: w666 -> [w704]
          tunnel: w659 -> [w703]
          tunnel: w662 -> [w694] mode=indexing
          tunnel: w661 -> [w699]
          tunnel: w654 -> [w693]
          shift-right: [w681] -> w658
          shift-left: 0 -> [w680]
          tunnel: w657 -> [w677]
          tunnel: w648 -> [w676] mode=indexing
          i -> [w710]
          w685 = i16 1 ("left")
          n349 = Unbundle By Name(w676) -> ("Item"=w700:string, "Options"=w702:string[], "Icons"=w695:T19[])
          n350 = Multiply(x=w710, y=w711) -> (x*y=w713:i32)
          n351 = Increment(x=w710) -> (x+1=w683:i32)
          n352 = Add(x=w699, y=w713) -> (x+y=w682:i32)
          n353 = Index Array(array=w702, index=w694) -> (element=w701:string)
          n354 = Index Array(array=w695, index=w694) -> (element=w692:T19)
          n355 = Decrement(x=w682) -> (x-1=w698:i32)
          n356 = Bundle By Name(cluster=cluster{"x":i16, "y":i16} {"x"=10, "y"=0} ("origin"), "x"=w705, "y"=w682) -> (w720:cluster{"x":i16, "y":i16})
          n357 = call <vilib>:"Draw Text at Point.vi"("[user-specified font]"=w707, "desired font(Application)"=w708, "text"=w700, "origin"=w720, "picture"=w723) -> ("text rect"=w679:T25, "new picture"=w721:picture)  [unwired: 5 in]
          n358 = Unbundle By Name(w716) -> ("Rectangle"=w717:T25)
          n359 = Unbundle By Name(w679) -> ("bottom"=w678:i16)
          n360 = Bundle By Name(cluster=w720, "x"=w704) -> (w719:cluster{"x":i16, "y":i16})
          n361 = Bundle(cluster=T25 {"left"=0, "top"=0, "right"=0, "bottom"=0} ("y"), "left"=w703, "top"=w698, "right"=w703, "bottom"=w698) -> (w687:T25)
          n362 = Bundle(cluster=w687, "left"=w685, "right"=w685) -> (w686:T25)  [unwired: 2 in]
          n363 = Add(x=w717, y=w687) -> (x+y=w712:T25)
          n364 = Bundle(cluster=w712, "left"=w704) -> (w709:T25)  [unwired: 3 in]
          n365 = Index Array(array=w693, index=w692) -> (element=w690:T17)
          n366 = call <vilib>:"Draw Text at Point.vi"("[user-specified font]"=w706, "desired font(Application)"=w708, "text"=w701, "origin"=w719, "picture"=w721) -> ("new picture"=w718:picture)  [unwired: 5 in, 1 out]
          n367 = Unbundle By Name(w690) -> ("Rectangle"=w689:T25)
          n368 = Bundle By Name(cluster=w716, "Rectangle"=w712) -> (w715:T17)
          n369 = Add(x=w689, y=w686) -> (x+y=w688:T25)
          n370 = Bundle By Name(cluster=w690, "Rectangle"=w688) -> (w691:T17)
          n371 = call <vilib>:"Draw Flattened Pixmap.vi"("image data"=w715, "picture"=w718) -> ("new picture"=w697:picture)  [unwired: 7 in]
          n372 = Less Or Equal?(x=w678, y=w677) -> (x <= y?=w684:bool)
          n373 = Select(t=w683, s=w684, f=w680) -> (s? t:f=w681:i32)
          n374 = call <vilib>:"Draw Flattened Pixmap.vi"("image data"=w691, "picture"=w697) -> ("new picture"=w696:picture)  [unwired: 7 in]
        }
        "Picture" <- w655
        n375 = Bundle By Name(cluster=w649, "MissingTypes.Rectangles"=w670, "MissingTypes.VerticalRows"=w658) -> (w656:T20)
      }
      frame "Missing:CheckScrollPos" {
        n376 = property on="Picture" class="Pict"() -> ("Top"=w726:i16)  [unwired: 2 in, 2 out]
        n377 = Unbundle By Name(w725) -> ("MissingTypes.Y-Distance"=w727:i32)
        n378 = Quotient & Remainder(x=w726, y=w727) -> (x-y*floor(x/y)=w733:i32, floor(x/y)=w730:i32)
        n379 = Divide(x=w727, y=2) -> (x/y=w732:dbl)
        n380 = Greater Or Equal?(x=w733, y=w732) -> (x >= y?=w731:bool)
        n381 = Increment(x=w730) -> (x+1=w729:i32)
        n382 = Select(t=w729, s=w731, f=w730) -> (s? t:f=w728:i32)
        n383 = Multiply(x=w728, y=w727) -> (x*y=w735:i32)
        n384 = property on="Picture" class="Pict"("Top"=w735) -> ()  [unwired: 2 in, 2 out]
        n385 = Bundle By Name(cluster=w725, "MissingTypes.IndexOffset"=w728) -> (w724:T20)
      }
      frame "Missing:ShowRing" {
        n386 = Unbundle By Name(w739) -> ("InterfaceItems"=w741:T18[], "Interface"=w742:bool, "MissingItems"=w740:T18[])
        n387 = property on="Picture" class="Pict"() -> ("Draw Area Size"=w760:T26)  [unwired: 2 in, 2 out]
        n388 = Select(t=w741, s=w742, f=w740) -> (s? t:f=w738:T18[])
        n389 = Unbundle By Name(w739) -> ("MissingTypes.YStart"=w747:i32, "MissingTypes.Rectangle"=w769:T25, "MissingTypes.IndexOffset"=w768:i32, "MissingTypes.Y-Distance"=w761:i32, "MissingTypes.XStart2"=w756:i32)
        n390 = Unbundle By Name(w739) -> ("MissingTypes.Row"=w751:i32, "MissingTypes.Selected"=w752:i32[])
        n391 = Unbundle By Name(w760) -> ("Width"=w759:u32)
        n392 = Index Array(array=w738, index=w751) -> (element=w763:T18)
        n393 = Index Array(array=w752, index=w751) -> (element=w750:i32)
        n394 = Add(x=w759, y=u32 3) -> (x+y=w757:u32)
        n395 = Subtract(x=w757, y=w756) -> (x-y=w754:u32)
        n396 = Unbundle By Name(w763) -> ("Options"=w762:string[])
        n397 = Unbundle By Name(w769) -> ("left"=w773:i16, "top"=w771:i16)
        n398 = property on="Picture" class="Pict"() -> ("MasterRect"=w775:T33)  [unwired: 2 in, 2 out]
        n399 = Multiply(x=w768, y=w761) -> (x*y=w766:i32)
        n400 = Unbundle By Name(w775) -> ("Left"=w774:i16, "Top"=w772:i16)
        n401 = Bundle(cluster=T26 {"Width"=93, "Height"=17} ("Named Numeric Size"), "Width"=w754) -> (w753:T26)  [unwired: 1 in]
        n402 = Add(x=w774, y=w773) -> (x+y=w765:i16)
        n403 = Add(x=w772, y=w771) -> (x+y=w767:i16)
        n404 = Subtract(x=w747, y=2 ("x")) -> (x-y=w746:i32)
        n405 = Decrement(x=w765) -> (x-1=w764:i16)
        n406 = Subtract(x=w767, y=w766) -> (x-y=w749:i32)
        n407 = Add(x=w749, y=w746) -> (x+y=w748:i32)
        n408 = property on="Ring" class="Ring (strict)"("Strings []"=w762, "Value"=w750, "Left"=w764, "Top"=w748, "NmdNumSize"=w753, "Visible"=TRUE ("ShowRing")) -> ()  [unwired: 2 in, 2 out]
        n409 = Bundle By Name(cluster=w739, "MissingTypes.ShowRing"=TRUE ("ShowRing")) -> (w744:T20)
      }
      frame "Missing:HideRing" {
        n410 = Bundle By Name(cluster=w778, "MissingTypes.ShowRing"=FALSE ("ShowRing")) -> (w779:T20)
        n411 = property on="Ring" class="Ring (strict)"("Visible"=FALSE ("ShowRing")) -> ()  [unwired: 2 in, 2 out]
      }
      frame "Missing:EnableNext?" {
        n412 = Unbundle By Name(w784) -> ("MissingTypes.Selected"=w792:i32[])  [unwired: 1 out]
        n413 = Unbundle By Name(w784) -> ("InterfaceItems"=w786:T18[], "Interface"=w787:bool, "MissingItems"=w785:T18[])
        n414 = Select(t=w786, s=w787, f=w785) -> (s? t:f=w783:T18[])
        n415 = for {
          tunnel: w792 -> [w797] mode=indexing
          tunnel: w783 -> [w799] mode=indexing
          tunnel: [w794] -> w789
          stop <- w794 stop-if-true
          n416 = Unbundle By Name(w799) -> ("Icons"=w798:T19[])
          n417 = Index Array(array=w798, index=w797) -> (element=w796:T19)
          n418 = Equal?(x=w796, y=ConvertTextBasedCodeToLabVIEW_MissingTypeIconType."?") -> (x = y?=w794:bool)
        }
        n419 = Select(t=T22."Disabled and Grayed Out" ("Disabled"), s=w789, f=T22."Enabled" ("Disabled")) -> (s? t:f=w790:T22)
        n420 = property on="Next" class="Bool"("DisabledEnum"=w790) -> ()  [unwired: 2 in, 2 out]
      }
      frame "------------------------" {
      }
      frame "CheckFiles" {
        n421 = Unbundle By Name(w805) -> ("Files"=w807:path[])
        n422 = for {
          tunnel: w807 -> [w810] mode=indexing
          shift-right: [w809] -> w804
          shift-left: path[] [] -> [w811]
          n423 = Search 1D Array(1D array=w811, element=w810) -> (index of element=w812:i32)  [unwired: 1 in]
          n424 = case shown="-1" w812 {
            tunnel: w811 -> [w813 w816]
            tunnel: w810 -> [_ w815]
            tunnel: [w813 w814] -> w809
            frame 0, Default {
            }
            frame -1 {
              n425 = Build Array (concatenate)(w816, w815) -> (w814:path[])
            }
          }
        }
        n426 = Bundle By Name(cluster=w805, "Files"=w804) -> (w803:T20)
      }
      frame "Summary" {
        # "Interfaces supported"
        n427 = Unbundle By Name(w830) -> ("InterfaceSelected"=w820:i32[], "InterfaceItems"=w822:T18[], "MissingItems"=w824:T18[], "Classes"=w819:T1[])
        n428 = Temporary Directory() -> (w832:path)
        n429 = disable-structure shown="Disabled" {
          disable-tunnel: w822 -> [w836 _]
          disable-tunnel: [w835 _] -> w821
          disable-tunnel: w820 -> [w834 _]
          frame Disabled {
            n430 = for {
              tunnel: w836 -> [w841] mode=indexing
              tunnel: [w840] -> w835 mode=indexing if=w837
              tunnel: w834 -> [w839] mode=indexing
              n431 = Unbundle By Name(w841) -> ("Item"=w840:string)
              n432 = Equal?(x=w839, y=1) -> (x = y?=w837:bool)
            }
          }
          frame Enabled {
          }
        }
        n433 = Build Path(base path=w832, name or relative path="ConvertTextToLV_Overview.html") -> (appended path=w829:path)
        n434 = for {
          tunnel: w824 -> [w846] mode=indexing
          tunnel: [w845] -> w823 mode=indexing
          n435 = Unbundle By Name(w846) -> ("Item"=w845:string)
        }
        n436 = local read "BetterNames"() -> (w817:bool)
        n437 = case shown="True" w817 {
          tunnel: w819 -> [w842 w844]
          tunnel: [w842 w843] -> w818
          frame False {
          }
          frame True {
            n438 = call "ConvertTextBasedCodeToLabVIEW_MakenamesBetter.vi"("ClassesIn"=w844) -> ("ClassesOut"=w843:T1[])  [unwired: 10 in]
          }
        }
        n439 = call "ConvertTextBasedCodeToLabVIEW_CreateOverviewHtmlFile.vi"("InterfacesThatWillUseInheritance"=w821, "MissingClasses"=w823, "error in (no error)"=w826, "Classes"=w818, "appended path in"=w829) -> ("error out"=w827:errorcluster, "appended path out"=w828:path)  [unwired: 5 in]
        n440 = call-poly <vilib>:"Open URL in Default Browser.vi"("error in (no error)"=w827, "path"=w828) -> ("error out"=w825:errorcluster)  [unwired: 4 in, 1 out]
      }
      frame "CreateClasses" {
        w858 = FALSE ("Visible")
        n441 = Unbundle By Name(w870) -> ("InterfaceSelected"=w849:i32[], "InterfaceItems"=w850:T18[], "MissingTypeSelected"=w864:i32[], "Classes"=w869:T1[], "MissingItems"=w863:T18[], "ExistingClassesFolders"=w868:path[], "StructsOusideClass"=w854:T12[], "EnumsOusideClass"=w853:T11[])
        n442 = local read "ClassType"() -> (w861:T14)
        n443 = local read "Top Folder for all classes"() -> (w867:path)
        n444 = property on="Tab" class="TabCtl (strict)"("Value"=T13."Working" ("Tab")) -> ()  [unwired: 2 in, 2 out]
        n445 = case shown="\"Reference Object  (GOOP3)\"" w861 {
          tunnel: [GDSAPI_ClassProviderType."LabVIEW Native(By value)" ("ClassProvider") GDSAPI_ClassProviderType."GOOP-4(By reference)" ("ClassProvider") GDSAPI_ClassProviderType."GOOP-3(By reference)" ("ClassProvider")] -> w855
          frame "Native By Value LabVIEW Classes", Default {
          }
          frame "Reference Object DVR (GOOP4)" {
          }
          frame "Reference Object  (GOOP3)" {
          }
        }
        n446 = for {
          tunnel: w863 -> [w882] mode=indexing
          tunnel: w864 -> [w881] mode=indexing
          tunnel: [w880] -> w862 mode=indexing
          n447 = Bundle By Name(cluster=w882, "Index"=w881) -> (w880:T18)
        }
        n448 = property on="Previous" class="Bool"("Visible"=w858) -> ()  [unwired: 2 in, 2 out]
        n449 = property on="Next" class="Bool"("Visible"=w858) -> ()  [unwired: 2 in, 2 out]
        n450 = control-ref of="ProgressText"() -> (w859:refnum<vi>)
        n451 = for {
          tunnel: w850 -> [w876] mode=indexing
          tunnel: [w875] -> w848 mode=indexing if=w872
          tunnel: w849 -> [w874] mode=indexing
          n452 = Unbundle By Name(w876) -> ("Item"=w875:string)
          n453 = Equal?(x=w874, y=1) -> (x = y?=w872:bool)
        }
        n454 = Bundle By Name(cluster=T27 {"ClassProvider"=enum."GOOP-4(By reference)", "PropertyMethodType"=enum."PropertyMethod", "Pattern type"=0} ("Options"), "ClassProvider"=w855, "PropertyMethodType"="PropertyMethodType", "Pattern type"="VI/Method Pattern type") -> (w856:T27)
        n455 = call "ConvertTextBasedCodeToLabVIEW_CreateClasses.vi"("Classes"=w869, "TopFolder"=w867, "InterfacesThatShouldBeConvertedToClasses"=w848, "Options"=w856, "MissingItems"=w862, "BetterNames"="BetterNames", "ExistingClassFolders"=w868, "error in (no error)"=w866, "ProgressTextRef"=w859, "StructsOusideClass"=w854, "EnumsOusideClass"=w853) -> ("error out"=w865:errorcluster)  [unwired: 4 in]
      }
      frame "Done" {
        n456 = Two Button Dialog(message="Conversion done.", 1:"Quit" ("F button name (\"Cancel\")"), 2:"Convert some more..." ("T button name (\"OK\")")) -> (T button?=w885:bool)
        n457 = Select(t="Init", s=w885, f="Exit") -> (s? t:f=w883:string)
      }
    }
    n458 = Equal?(x=w46, y="Exit") -> (x = y?=w49:bool)
    n459 = Select(t="Error", s=w45, f=w46) -> (s? t:f=w50:string)
  }
  "error IO" <- w13
  n460 = stacked-sequence {
    tunnel: w13 -> [_]
    frame #0 {
      n461 = invoke class="VI" method="FP.Close"() -> ()  [unwired: 3 in, 3 out]
      n462 = property on="Ring" class="Ring (strict)"("Visible"=TRUE ("ShowRing")) -> ()  [unwired: 2 in, 2 out]
      n463 = property on="Ring" class="Ring (strict)"("Position"=T34 {"Left"=-149, "Top"=45}) -> ()  [unwired: 2 in, 2 out]
    }
  }
  "MissingText1" <- w5
  "MissingText2" <- w4
